vi "Gestion regulateurs EUROTHERM EPC3000.vi"() -> ()   [LabVIEW 2022 SP3]
uses:
  Enum/Enum r14.ctl
  Enum/Enum r7.ctl
  Variables globales/Variable glob generale.vi
  Variables globales/Variables glob EUROTHERM.vi
panel:
  in  "Onglets port COM":T1(tab)
  in  "1 COM reg":T2(array[cluster]) caption="COM1"
  in  "1 COM reg 2":T2(array[cluster])
  in  "1 COM reg 3":T2(array[cluster])
  in  "1 COM reg 4":T2(array[cluster])
  in  "1 COM reg 5":T2(array[cluster])
  out "Action":string="\nAction en cours\nVeuillez patienter"
  out "référence en sortie":refnum<vi>
  out "CUVE":string
  out "Fichier de rapport":path caption="Fichier rapport"
  out "Listing programmes":string
  out "Config + programmes":T3
  in  "Onglets actions":T4(tab)
  in  "Envoyer profil":bool
  in  "Onglet_Tinit":enum32{"Définir Tinit", "Acquérir Tinit"}(tab)
  in  "Val T ini":dbl=20.0 format="%#.1f"
  in  "Régulateur":u16(ring) items=["avant", "centre", "arrière"]
  in  "Début du profil":timestamp format="%<%H:%M:%S\n%A %d/%m/%y>T"
  in  "Charger profil":bool
  in  "Lire régulateur":bool
  in  "Sauvegarder profil":bool
  in  "Stop Régulation":bool
  in  "Start Régulation":bool
  in  "Test surveillance reg":bool caption="Accès par mot de passe"
  in  "Lire les alarmes":bool
  in  "Modifier les alarmes":bool
  in  "Alarme haute":dbl caption="Alarme haute (°C)" format="%#.1f"
  in  "Alarme basse":dbl caption="Alarme basse (°C)" format="%#.1f"
  in  "stop":bool
  out "Profil":cluster{"Y":dbl[], "Y":dbl[]}[](graph)
  out "Type de fin":string
  # "gestion des régulateurs EPC3000\n(PROTOCOLE MODBUS)"
  # "Ce logiciel et les informations qu'il contient, sont la propriété de l’IAS et ne peuvent être diffusés sans l’autorisation de la Station d’étalonnage"
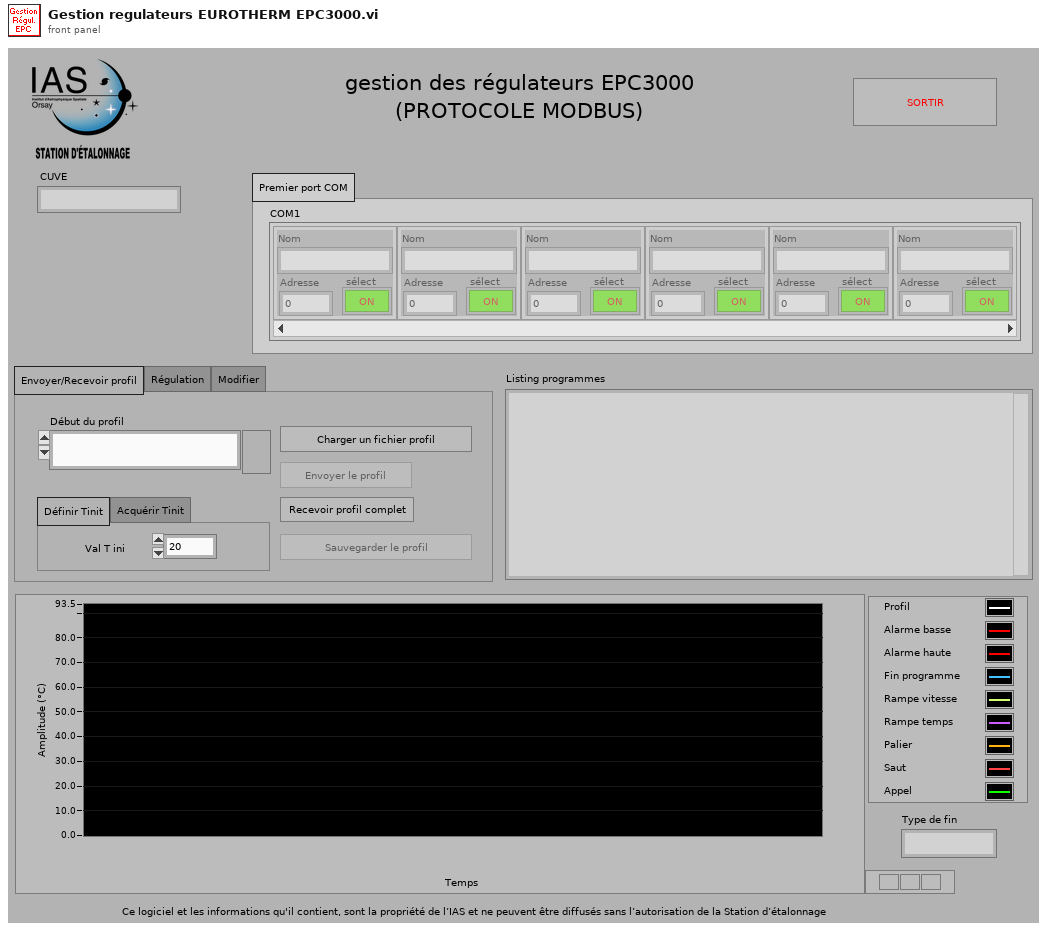
[diagram p1: front panel]
types:
  T1 = enum32{"Premier port COM", "Deuxième port COM", "Troisième port COM", "Quatrième port COM", "Cinquième port COM"}
  T2 = cluster{"Nom":string, "Adresse":u8, "sélect":bool}[]
  T3 = cluster{"config":cluster{"key":string, "value":dbl}[], "Prog 1 en sortie":cluster{string, dbl}[][], "Prog 2 en sortie":cluster{string, dbl}[][], "Prog 3 en sortie":cluster{string, dbl}[][], "Prog 4 en sortie":cluster{string, dbl}[][], "Prog 5 en sortie":cluster{string, dbl}[][], "Prog 6 en sortie":cluster{string, dbl}[][], "Prog 7 en sortie":cluster{string, dbl}[][], "Prog 8 en sortie":cluster{string, dbl}[][], "Prog 9 en sortie":cluster{string, dbl}[][], "Prog 10 en sortie":cluster{string, dbl}[][]}
  T4 = enum32{"Envoyer/Recevoir profil", "Régulation", "Modifier"}
  T5 = enum32{"Invalid", "Standard", "Closed", "Hidden", "Minimized", "Maximized"}
  T6 = cluster{cluster{"key":string, "value":i32}[], "Programme en sortie":cluster{string, dbl}[][], "Programme en sortie":cluster{string, dbl}[][], "Programme en sortie":cluster{string, dbl}[][], "Programme en sortie":cluster{string, dbl}[][], "Programme en sortie 2":cluster{string, dbl}[][], "Programme en sortie 3":cluster{string, dbl}[][], "Programme en sortie 4":cluster{string, dbl}[][], "Programme en sortie 5":cluster{string, dbl}[][], "Programme en sortie 6":cluster{string, dbl}[][], "Programme en sortie 7":cluster{string, dbl}[][]}
  T7 = enum8{"Enabled", "Disabled", "Disabled and Grayed Out"}
  T8 = typedef "Enum r14.ctl" = enum16{"RUN ?", "Arrêter ?", "Arrêt", "envoi profil", "fin"}
  T9 = typedef "Enum r7.ctl" = enum16{"validation liste", "réception profils", "validation RUN", "fin"}
  T10 = cluster{"1 COM reg":cluster{"Nom":string, "Adresse":u8, "sélect":bool}[]}[]
  T11 = cluster{"1 COM reg":cluster{"Nom":string, "Adresse":u8, "sélect":bool}[]}
  T12 = cluster{"config":cluster{"key":string, "value":dbl}[], "Prog 1":cluster{string, dbl}[][], "Prog 2":cluster{string, dbl}[][], "Prog 3":cluster{string, dbl}[][], "Prog 4":cluster{string, dbl}[][], "Prog 5":cluster{string, dbl}[][], "Prog 6":cluster{string, dbl}[][], "Prog 7":cluster{string, dbl}[][], "Prog 8":cluster{string, dbl}[][], "Prog 9":cluster{string, dbl}[][], "Prog 10":cluster{string, dbl}[][]}
  T13 = cluster{"Tempé. max":dbl, "Tempé. min":dbl, "Temps max":dbl, "Temps min":dbl}
  T14 = cluster{"Noms voies select acqui 1COM":string[]}[]
  T15 = cluster{"Ev_Saut":dbl[], "Ev_Palier":dbl[], "Ev_Rampe_vitesse":dbl[], "Ev_Rampe_temps":dbl[], "Ev_Appel":dbl[], "Ev_Fin":dbl[], "T_Fin":dbl[], "T_Appel":dbl[], "T_Rampe_temps":dbl[], "T_Rampe_vitesse":dbl[], "T_Palier":dbl[], "T_Saut":dbl[], "Type de fin":string}
  T16 = typedef "Commande Choix arret reg.ctl" = u16
  T17 = cluster{"Programmation configuration":cluster{"Command (PV)":string, dbl}[], "Programme 1":cluster{"chaîne o":string, "Received Value":dbl}[][], "Programme 2":cluster{"chaîne o":string, "Received Value":dbl}[][], "Programme 3":cluster{"chaîne o":string, "Received Value":dbl}[][], "Programme 4":cluster{"chaîne o":string, "Received Value":dbl}[][], "Programme 5":cluster{"chaîne o":string, "Received Value":dbl}[][], "Programme 6":cluster{"chaîne o":string, "Received Value":dbl}[][], "Programme 7":cluster{"chaîne o":string, "Received Value":dbl}[][], "Programme 8":cluster{"chaîne o":string, "Received Value":dbl}[][], "Programme 9":cluster{"chaîne o":string, "Received Value":dbl}[][], "Programme 10":cluster{"chaîne o":string, "Received Value":dbl}[][]}
  T18 = cluster{"config":cluster{"key":string, "value":dbl}[], "Programme_sortie":cluster{"chaîne":string, "Valeur":dbl}[][], "Programme_sortie":cluster{"chaîne":string, "Valeur":dbl}[][], "Programme_sortie":cluster{"chaîne":string, "Valeur":dbl}[][], "Programme_sortie":cluster{"chaîne":string, "Valeur":dbl}[][], "Programme_sortie":cluster{"chaîne":string, "Valeur":dbl}[][], "Programme_sortie":cluster{"chaîne":string, "Valeur":dbl}[][], "Programme_sortie":cluster{"chaîne":string, "Valeur":dbl}[][], "Programme_sortie":cluster{"chaîne":string, "Valeur":dbl}[][], "Programme_sortie":cluster{"chaîne":string, "Valeur":dbl}[][], "Programme_sortie":cluster{"chaîne":string, "Valeur":dbl}[][]}
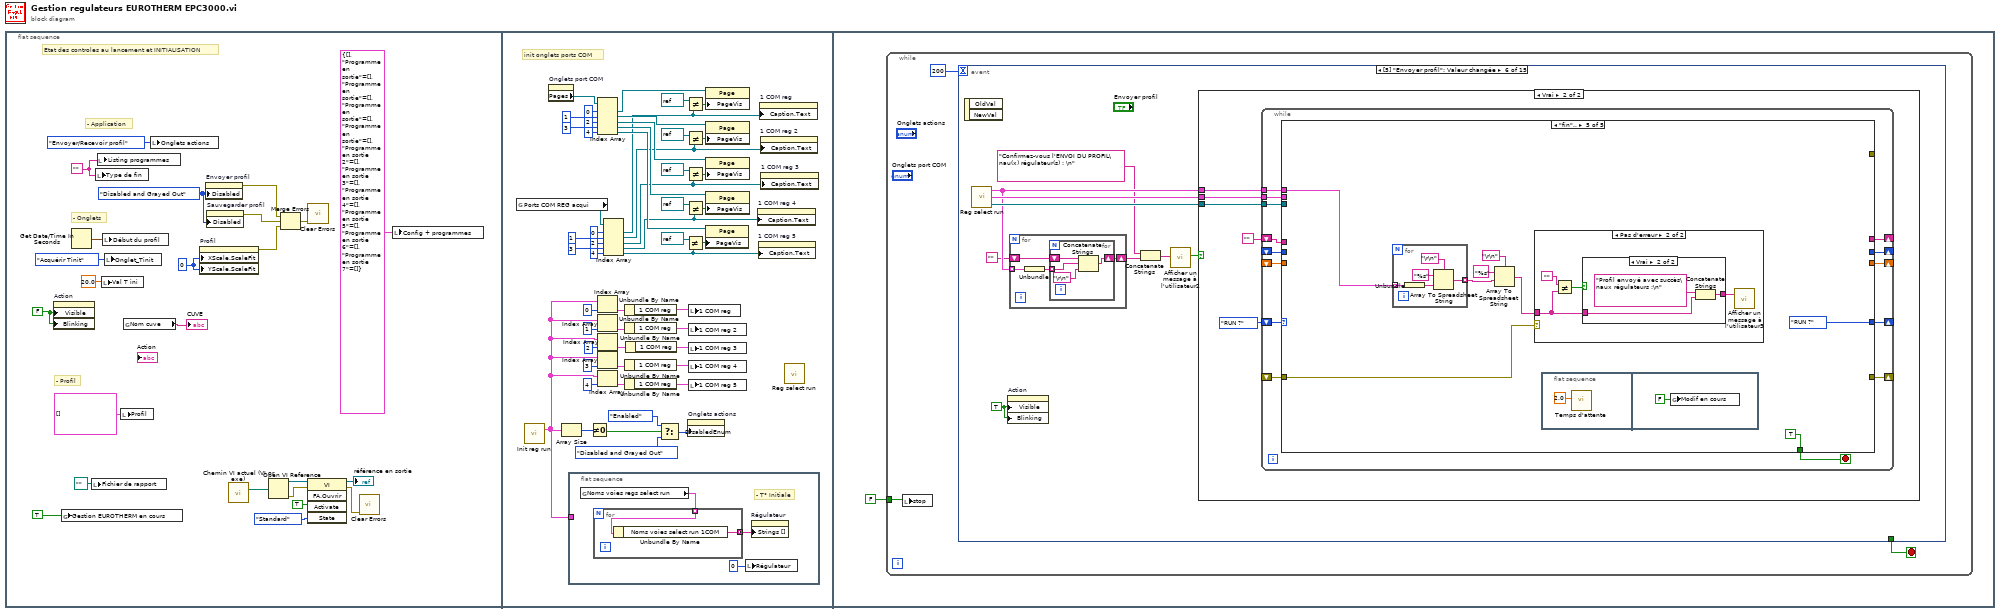
[diagram p0: block diagram]
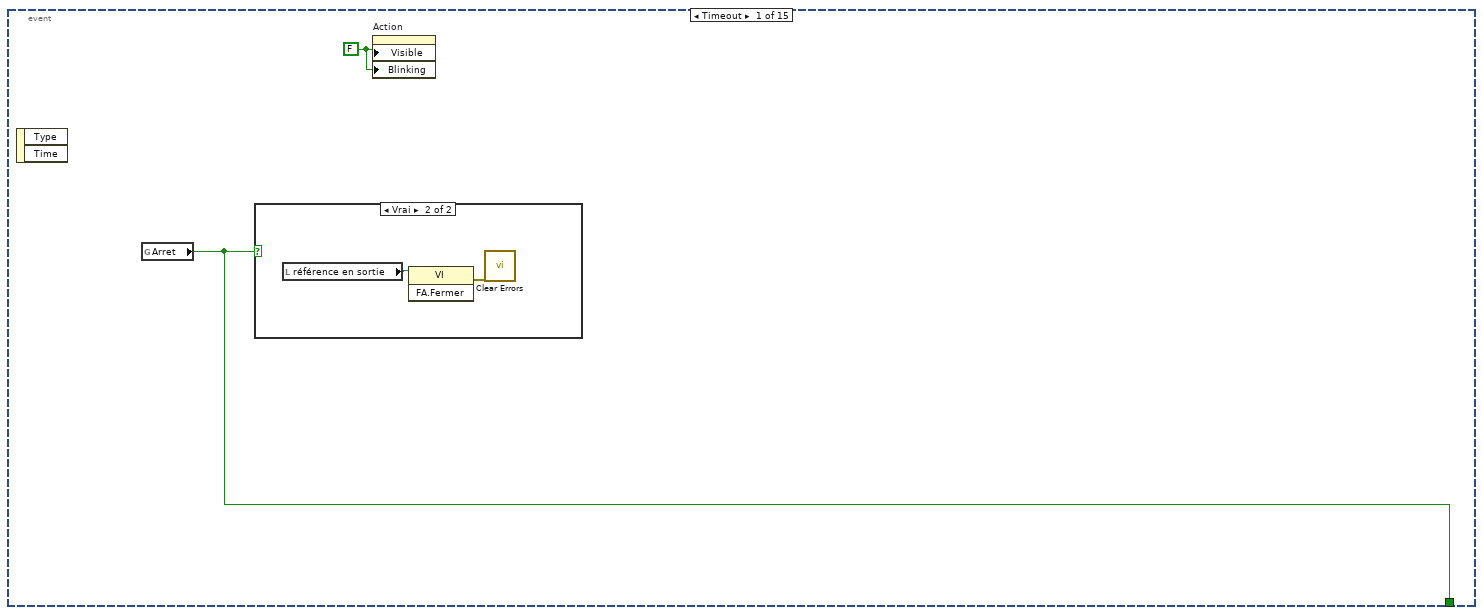
[diagram p2: hidden frame]
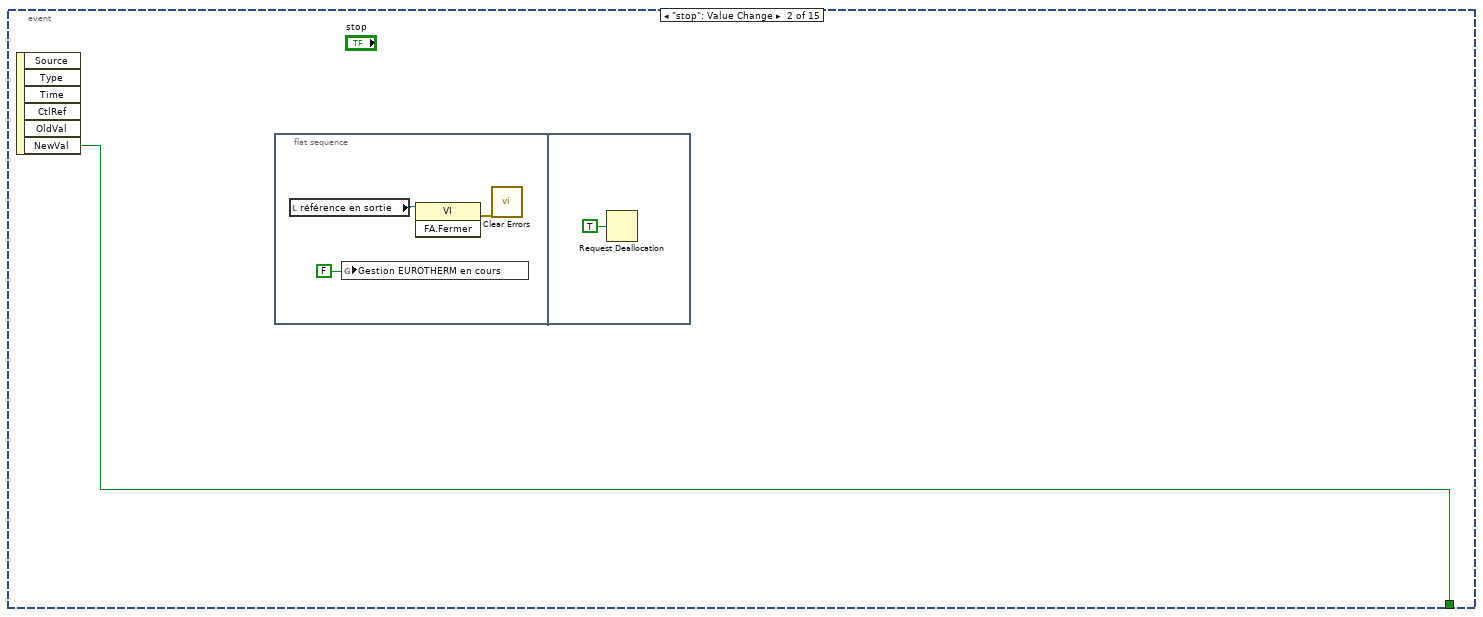
[diagram p4: hidden frame]
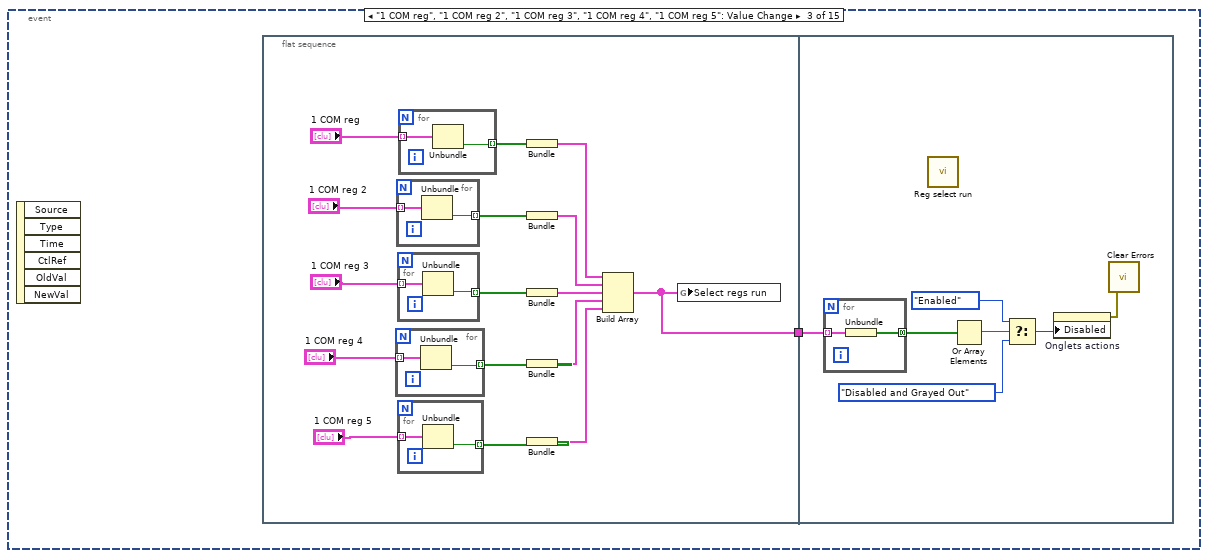
[diagram p5: hidden frame]
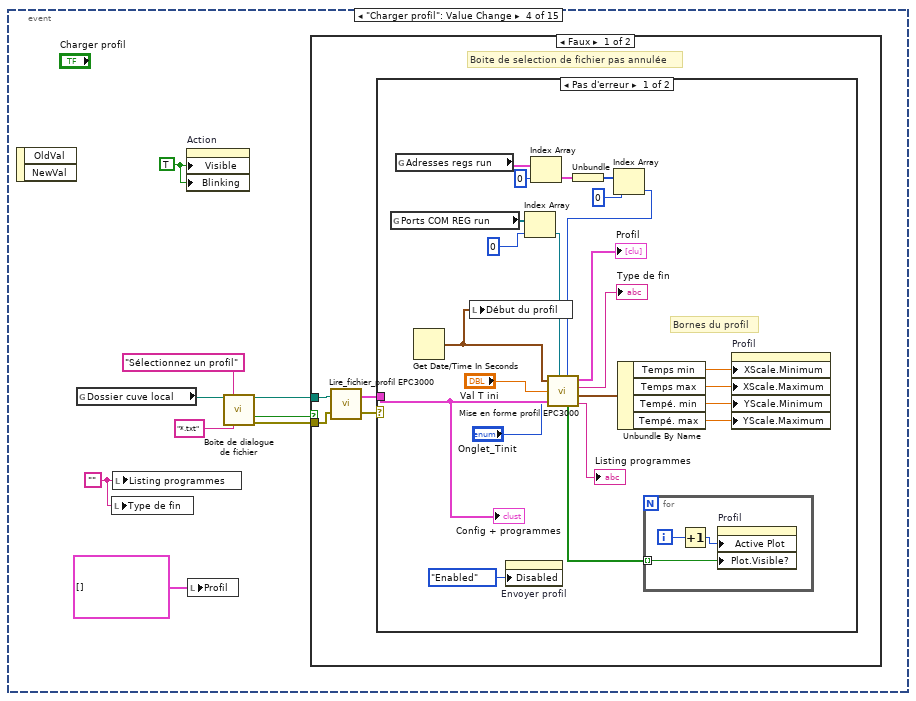
[diagram p6: hidden frame]
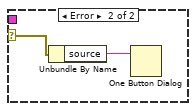
[diagram p7: hidden frame]
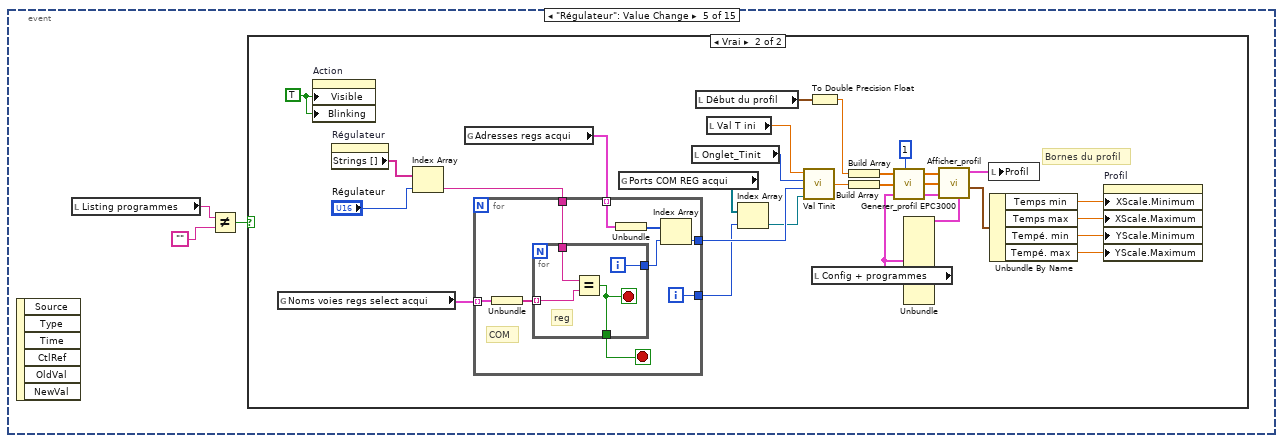
[diagram p9: hidden frame]
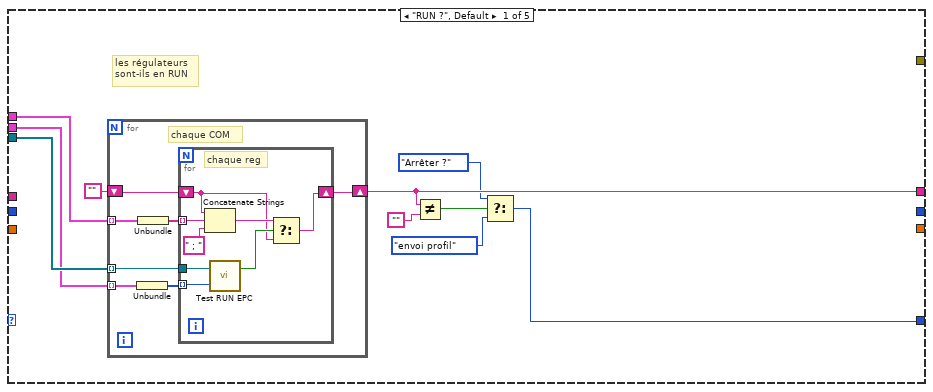
[diagram p12: hidden frame]
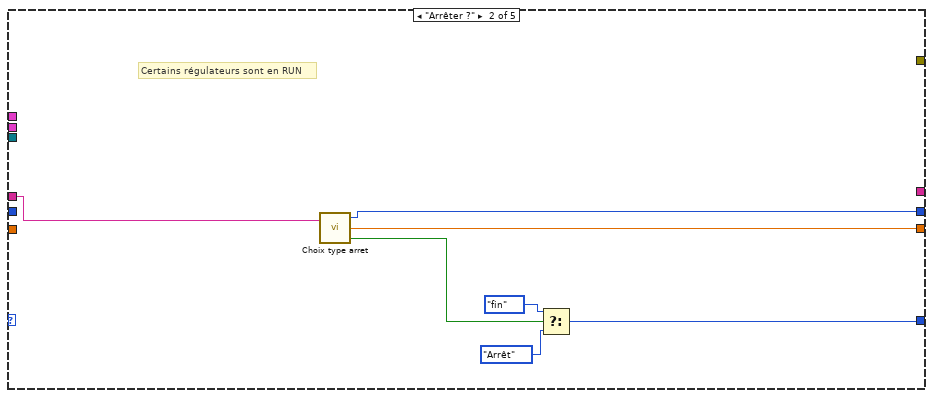
[diagram p13: hidden frame]
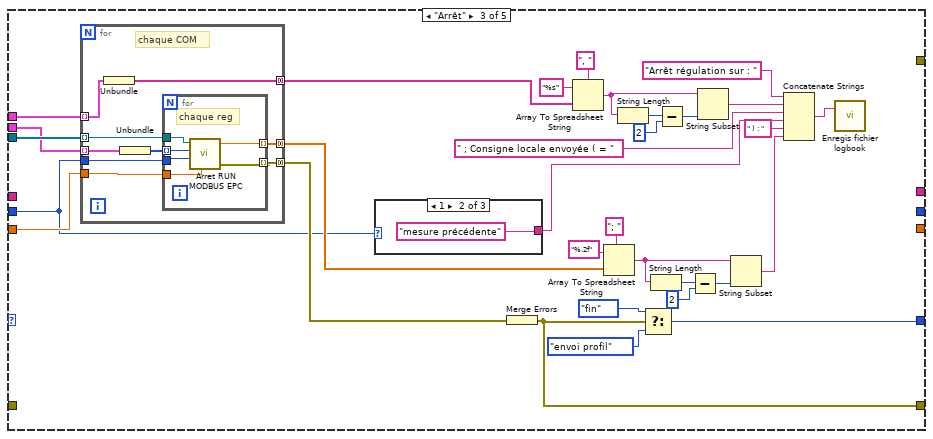
[diagram p14: hidden frame]
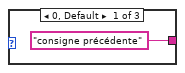
[diagram p15: hidden frame]
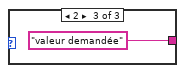
[diagram p16: hidden frame]
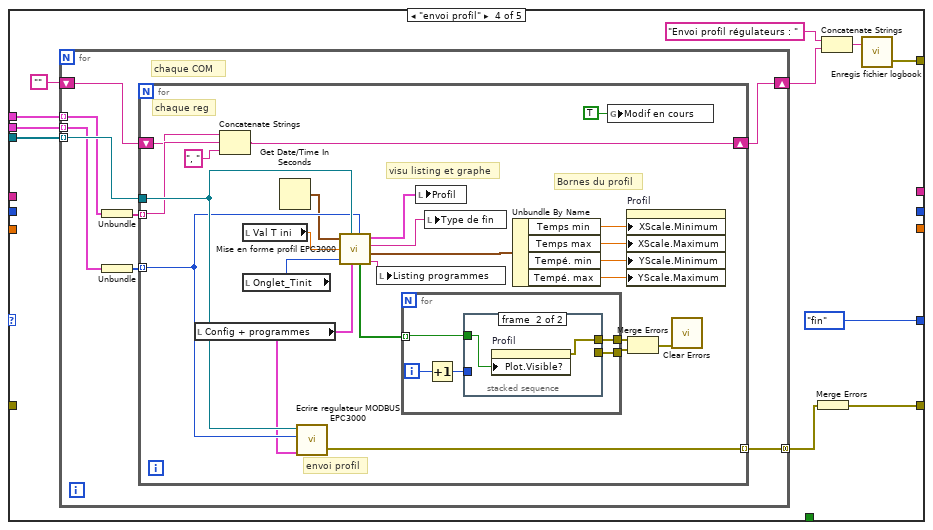
[diagram p17: hidden frame]
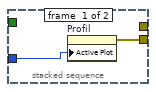
[diagram p18: hidden frame]
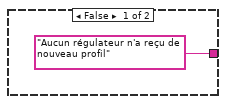
[diagram p20: hidden frame]
diagram:
  n1 = flat-sequence {
    frame #0 {
      w2 = T7."Disabled and Grayed Out" ("Désactivé")
      w3 = FALSE ("Visible")
      w22 = u8 0 ("Échelle des X.Ajuster l'échelle")
      w24 = ""
      # "- Onglets"
      # "- Profil"
      # "- Application"
      # "Etat des controles au lancement et INITIALISATION"
      n2 = property on="Action" class="Ch"("Visible"=w3, "Blinking"=w3) -> ()  [unwired: 2 in, 2 out]
      n3 = global write "Variable glob generale.vi" "Gestion EUROTHERM en cours"(TRUE ("Gestion reg en cours")) -> ()
      n4 = Get Date/Time In Seconds() -> (seconds since 1Jan1904=w21:timestamp)
      n5 = local write "Fichier de rapport"(path "" ("Fichier de rapport")) -> ()
      n6 = local write "Type de fin"(w24) -> ()
      n7 = local write "Listing programmes"(w24) -> ()
      n8 = local write "Val T ini"(20.0 ("Val_Tinit")) -> ()
      n9 = local write "Début du profil"(w21) -> ()
      n10 = local write "Onglet_Tinit"(enum32{"Définir Tinit", "Acquérir Tinit"}."Acquérir Tinit" ("Onglet_Tinit")) -> ()
      n11 = local write "Profil"(cluster{"Y":dbl[], "Y":dbl[]}[] [] ("Profil")) -> ()
      n12 = global read "Variable glob generale.vi" "Nom cuve"() -> (→"CUVE":string)
      n13 = local write "Onglets actions"(T4."Envoyer/Recevoir profil" ("Onglets actions")) -> ()
      n14 = property on="Profil" class="GraphXY (strict)"("XScale.ScaleFit"=w22, "YScale.ScaleFit"=w22) -> (error out=w15:errorcluster)  [unwired: 2 in, 1 out]
      n15 = property on="Envoyer profil" class="Bool"("Disabled"=w2) -> (error out=w16:errorcluster)  [unwired: 2 in, 1 out]
      n16 = property on="Sauvegarder profil" class="Bool"("Disabled"=w2) -> (error out=w14:errorcluster)  [unwired: 2 in, 1 out]
      n17 = call "Chemin VI actuel (VI or exe).vi"() -> ("Full Path to VI or executable"=w1:path)  [unwired: 14 in, 1 out]
      n18 = Open VI Reference(vi path=w1) -> (vi reference=w7:refnum<vi>, error out=w9:errorcluster)  [unwired: 5 in]
      n19 = Merge Errors(w16, w14, w15) -> (w13:errorcluster)
      n20 = invoke class="VI" method="FA.Ouvrir"(reference=w7, error in=w9, "Activate"=TRUE ("Activer ?"), "State"=T5."Standard" ("État")) -> (reference out=→"référence en sortie":refnum<vi>, error out=w10:errorcluster)  [unwired: 1 in, 3 out]
      n21 = call <vilib>:"Clear Errors.vi"("error in (no error)"=w13) -> ()  [unwired: 5 in, 2 out]
      n22 = call <vilib>:"Clear Errors.vi"("error in (no error)"=w10) -> ()  [unwired: 5 in, 2 out]
      n23 = local write "Config + programmes"(T6 {[], "Programme en sortie"=[], "Programme en sortie"=[], "Programme en sortie"=[], "Programme en sortie"=[], "Programme en sortie 2"=[], "Programme en sortie 3"=[], "Programme en sortie 4"=[], "Programme en sortie 5"=[], "Programme en sortie 6"=[], "Programme en sortie 7"=[]} ("Config + programmes")) -> ()
    }
    frame #1 {
      # "init onglets ports COM"
      n24 = global read "Variables glob EUROTHERM.vi" "Ports COM REG acqui"() -> (w65:refnum<visa-resource-name>[])
      n25 = call "Init reg run.vi"() -> ("Rég acqui"=w30:T10)  [unwired: 3 in]
      n26 = property on="Onglets port COM" class="Onglet (strict)"() -> ("Pages"=w72:refnum<vi>[])  [unwired: 2 in, 2 out]
      n27 = Array Size(array=w30) -> (size(s)=w29:i32)
      n28 = flat-sequence {
        tunnel: w30 -> [_]
        frame #0 {
          # "- T° Initiale"
          n29 = global read "Variables glob EUROTHERM.vi" "Noms voies regs select run"() -> (w80:cluster{"Noms voies select run 1COM":string[]}[])
          n30 = for {
            tunnel: w80 -> [w82] mode=indexing
            tunnel: [w81] -> w79 mode=concatenating
            n31 = Unbundle By Name(w82) -> ("Noms voies select run 1COM"=w81:string[])
          }
          n32 = local write "Régulateur"(0) -> ()
          n33 = property on="Régulateur" class="MDér (strict)"("Strings []"=w79) -> ()  [unwired: 2 in, 2 out]
        }
      }
      n34 = Not Equal To 0?(x=w29) -> (x != 0?=w28:bool)
      n35 = Index Array(array=w30, index=0 ("indice")) -> (element=w49:T11)
      n36 = Index Array(array=w30, index=1 ("indice")) -> (element=w46:T11)
      n37 = Index Array(array=w30, index=3 ("indice")) -> (element=w40:T11)
      n38 = Index Array(array=w30, index=4 ("indice")) -> (element=w37:T11)
      n39 = Index Array(array=w72, index #1=0 ("indice"), index #2=1 ("indice"), index #3=2 ("indice"), index #4=3 ("indice"), index #5=4 ("indice")) -> (element #1=w71:refnum<vi>, element #2=w60:refnum<vi>, element #3=w53:refnum<vi>, element #4=w52:refnum<vi>, element #5=w51:refnum<vi>)
      n40 = Index Array(array=w30, index=2 ("indice")) -> (element=w43:T11)
      n41 = Index Array(array=w65, index #1=0 ("indice"), index #2=1 ("indice"), index #3=2 ("indice"), index #4=3 ("indice"), index #5=4 ("indice")) -> (element #1=w33:refnum<visa-resource-name>, element #2=w32:refnum<visa-resource-name>, element #3=w31:refnum<visa-resource-name>, element #4=w34:refnum<visa-resource-name>, element #5=w35:refnum<visa-resource-name>)
      n42 = Unbundle By Name(w49) -> ("1 COM reg"=w48:T2)
      n43 = Unbundle By Name(w46) -> ("1 COM reg"=w47:T2)
      n44 = Unbundle By Name(w40) -> ("1 COM reg"=w41:T2)
      n45 = Unbundle By Name(w37) -> ("1 COM reg"=w36:T2)
      n46 = Unbundle By Name(w43) -> ("1 COM reg"=w42:T2)
      n47 = Select(t=T7."Enabled" ("Désactivé"), s=w28, f=T7."Disabled and Grayed Out" ("Désactivé")) -> (s? t:f=w25:T7)
      n48 = Not Equal?(x=refnum<visa-resource-name> refnum, y=w35) -> (x != y?=w54:bool)
      n49 = Not Equal?(x=refnum<visa-resource-name> refnum, y=w33) -> (x != y?=w64:bool)
      n50 = Not Equal?(x=refnum<visa-resource-name> refnum, y=w32) -> (x != y?=w61:bool)
      n51 = Not Equal?(x=refnum<visa-resource-name> refnum, y=w31) -> (x != y?=w56:bool)
      n52 = Not Equal?(x=refnum<visa-resource-name> refnum, y=w34) -> (x != y?=w59:bool)
      n53 = property on="Onglets actions" class="Onglet (strict)"("DisabledEnum"=w25) -> ()  [unwired: 2 in, 2 out]
      n54 = local write "1 COM reg"(w48) -> ()
      n55 = local write "1 COM reg 2"(w47) -> ()
      n56 = local write "1 COM reg 3"(w42) -> ()
      n57 = local write "1 COM reg 4"(w41) -> ()
      n58 = local write "1 COM reg 5"(w36) -> ()
      n59 = property class="Page"(reference=w51, "PageVis"=w54) -> ()  [unwired: 1 in, 2 out]
      n60 = property class="Page"(reference=w71, "PageVis"=w64) -> ()  [unwired: 1 in, 2 out]
      n61 = property class="Page"(reference=w60, "PageVis"=w61) -> ()  [unwired: 1 in, 2 out]
      n62 = property class="Page"(reference=w53, "PageVis"=w56) -> ()  [unwired: 1 in, 2 out]
      n63 = property class="Page"(reference=w52, "PageVis"=w59) -> ()  [unwired: 1 in, 2 out]
      n64 = property on="1 COM reg 4" class="Tabl (strict)"("Caption.Text"=w34) -> ()  [unwired: 2 in, 2 out]
      n65 = property on="1 COM reg 5" class="Tabl (strict)"("Caption.Text"=w35) -> ()  [unwired: 2 in, 2 out]
      n66 = property on="1 COM reg" class="Tabl (strict)"("Caption.Text"=w33) -> ()  [unwired: 2 in, 2 out]
      n67 = property on="1 COM reg 2" class="Tabl (strict)"("Caption.Text"=w32) -> ()  [unwired: 2 in, 2 out]
      n68 = property on="1 COM reg 3" class="Tabl (strict)"("Caption.Text"=w31) -> ()  [unwired: 2 in, 2 out]
      n69 = call "Reg select run.vi"() -> ()  [unwired: 2 in, 3 out]
    }
    frame #2 {
      n70 = while {
        tunnel: FALSE ("stop") -> [w86]
        stop <- w84 stop-if-true
        n71 = local write "stop"(w86) -> ()
        n72 = event shown="[5] \"Envoyer profil\": Valeur changée" {
          selector: _ -> [_ _ _ _ _ _ _ _ _ _ _ _ _ _ _]
          dyn-events: _ -> [_ _ _ _ _ _ _ _ _ _ _ _ _ _ _]
          timeout: 200 -> [_ _ _ _ _ _ _ _ _ _ _ _ _ _ _]
          tunnel: [w88 w91 _ _ _ _ _ _ _ _ _ _ _ _ _] -> w84
          event Timeout {
            w87 = FALSE ("Visible")
            n73 = event-data() -> ()  [unwired: 1 in, 2 out]
            n74 = global read "Variable glob generale.vi" "Arret"() -> (w88:bool)
            n75 = case shown="Vrai" w88 {
              frame False {
              }
              frame True {
                n76 = local read "référence en sortie"() -> (w89:refnum<vi>)
                n77 = invoke class="VI" method="FA.Fermer"(reference=w89) -> (error out=w90:errorcluster)  [unwired: 2 in, 2 out]
                n78 = call <vilib>:"Clear Errors.vi"("error in (no error)"=w90) -> ()  [unwired: 5 in, 2 out]
              }
            }
            n79 = property on="Action" class="Ch"("Visible"=w87, "Blinking"=w87) -> ()  [unwired: 2 in, 2 out]
          }
          event "stop": Value Change {
            n80 = event-data() -> ("NewVal"=w91:bool)  [unwired: 1 in, 5 out]
            n81 = flat-sequence {
              frame #0 {
                n82 = local read "référence en sortie"() -> (w93:refnum<vi>)
                n83 = global write "Variable glob generale.vi" "Gestion EUROTHERM en cours"(FALSE ("Gestion reg en cours")) -> ()
                n84 = invoke class="VI" method="FA.Fermer"(reference=w93) -> (error out=w94:errorcluster)  [unwired: 2 in, 2 out]
                n85 = call <vilib>:"Clear Errors.vi"("error in (no error)"=w94) -> ()  [unwired: 5 in, 2 out]
              }
              frame #1 {
                n86 = Request Deallocation(TRUE ("flag")) -> ()
              }
            }
          }
          event "1 COM reg", "1 COM reg 2", "1 COM reg 3", "1 COM reg 4", "1 COM reg 5": Value Change {
            n87 = event-data() -> ()  [unwired: 1 in, 6 out]
            n88 = flat-sequence {
              tunnel: [w97] -> w96
              tunnel: w96 -> [w123]
              frame #0 {
                n89 = for {
                  tunnel: "1 COM reg 4" -> [w116] mode=indexing
                  tunnel: [w115] -> w101 mode=indexing
                  n90 = Unbundle(w116) -> ("sélect"=w115:bool)  [unwired: 2 out]
                }
                n91 = for {
                  tunnel: "1 COM reg 2" -> [w120] mode=indexing
                  tunnel: [w119] -> w105 mode=indexing
                  n92 = Unbundle(w120) -> ("sélect"=w119:bool)  [unwired: 2 out]
                }
                n93 = for {
                  tunnel: "1 COM reg 3" -> [w118] mode=indexing
                  tunnel: [w117] -> w103 mode=indexing
                  n94 = Unbundle(w118) -> ("sélect"=w117:bool)  [unwired: 2 out]
                }
                n95 = for {
                  tunnel: "1 COM reg 5" -> [w114] mode=indexing
                  tunnel: [w113] -> w99 mode=indexing
                  n96 = Unbundle(w114) -> ("sélect"=w113:bool)  [unwired: 2 out]
                }
                n97 = for {
                  tunnel: "1 COM reg" -> [w122] mode=indexing
                  tunnel: [w121] -> w107 mode=indexing
                  n98 = Unbundle(w122) -> ("sélect"=w121:bool)  [unwired: 2 out]
                }
                n99 = Bundle(w107) -> (w106:cluster{bool[]})  [unwired: 1 in]
                n100 = Bundle(w105) -> (w104:cluster{bool[]})  [unwired: 1 in]
                n101 = Bundle(w103) -> (w102:cluster{bool[]})  [unwired: 1 in]
                n102 = Bundle(w101) -> (w100:cluster{bool[]})  [unwired: 1 in]
                n103 = Bundle(w99) -> (w98:cluster{bool[]})  [unwired: 1 in]
                n104 = Build Array(w106, w104, w102, w100, w98) -> (w97:cluster{bool[]}[])
                n105 = global write "Variables glob EUROTHERM.vi" "Select regs run"(w97) -> ()
              }
              frame #1 {
                n106 = for {
                  tunnel: w123 -> [w131] mode=indexing
                  tunnel: [w130] -> w124 mode=concatenating
                  n107 = Unbundle(w131) -> (w130:bool[])
                }
                n108 = call "Reg select run.vi"() -> ()  [unwired: 2 in, 3 out]
                n109 = Or Array Elements(Boolean array=w124) -> (logical OR=w127:bool)
                n110 = Select(t=T7."Enabled" ("Désactivé"), s=w127, f=T7."Disabled and Grayed Out" ("Désactivé")) -> (s? t:f=w129:T7)
                n111 = property on="Onglets actions" class="Onglet (strict)"("Disabled"=w129) -> (error out=w128:errorcluster)  [unwired: 2 in, 1 out]
                n112 = call <vilib>:"Clear Errors.vi"("error in (no error)"=w128) -> ()  [unwired: 5 in, 2 out]
              }
            }
          }
          event "Charger profil": Value Change {
            w133 = TRUE ("Visible")
            w134 = ""
            n113 = event-data() -> ()  [unwired: 1 in, 2 out]
            n114 = global read "Variable glob generale.vi" "Dossier cuve local"() -> (w136:path)
            n115 = local write "Type de fin"(w134) -> ()
            n116 = local write "Listing programmes"(w134) -> ()
            n117 = property on="Action" class="Ch"("Visible"=w133, "Blinking"=w133) -> ()  [unwired: 2 in, 2 out]
            n118 = local write "Profil"(cluster{"Y":dbl[], "Y":dbl[]}[] [] ("Profil")) -> ()
            n119 = call "Boîte de dialogue de fichier"("start path"=w136, "prompt"="Sélectionnez un profil", "pattern (all files)"="*.txt") -> ("selected path"=w137:path, "cancelled"=w138:bool, "error out"=w132:errorcluster)  [unwired: 9 in, 1 out]
            n120 = case shown="Faux" w138 {
              tunnel: w137 -> [w144 _]
              tunnel: w132 -> [w142 _]
              frame False {
                # "Boite de selection de fichier pas annulée"
                n121 = call "Lire_fichier_profil EPC3000.vi"("error in (no error)"=w142, "Chemin du fichier profil"=w144) -> ("error out"=w141:errorcluster, "Config + programmes"=w143:T12)
                n122 = case shown="Pas d'erreur" w141 {
                  selector: w141 -> [_ w172]
                  tunnel: w143 -> [w156 _]
                  frame No Error {
                    # "Bornes du profil"
                    n123 = global read "Variables glob EUROTHERM.vi" "Ports COM REG run"() -> (w153:refnum<visa-resource-name>[])
                    n124 = global read "Variables glob EUROTHERM.vi" "Adresses regs run"() -> (w150:cluster{"Adresses run 1COM reg":u16[]}[])
                    n125 = Get Date/Time In Seconds() -> (seconds since 1Jan1904=w154:timestamp)
                    n126 = local write "Début du profil"(w154) -> ()
                    n127 = property on="Envoyer profil" class="Bool"("Disabled"=T7."Enabled" ("Désactivé")) -> ()  [unwired: 2 in, 2 out]
                    n128 = Index Array(array=w153, index=0 ("indice")) -> (element=w151:refnum<visa-resource-name>)
                    n129 = Index Array(array=w150, index=0 ("indice")) -> (element=w148:cluster{"Adresses run 1COM reg":u16[]})
                    n130 = Unbundle(w148) -> ("Adresses run 1COM reg"=w147:u16[])
                    n131 = Index Array(array=w147, index=0 ("indice")) -> (element=w145:u16)
                    n132 = call "Mise en forme profil EPC3000.vi"("Début du profil"=w154, "Port COM run 1 REG"=w151, "Val T ini en entrée"="Val T ini", "Onglet_Tinit"="Onglet_Tinit", "Config + programmes"=w156, "adresse reg"=w145) -> ("Graphe XY"=→"Profil":cluster{"Y":dbl[], "Y":dbl[]}[], "Type de fin"=→"Type de fin":string, "Courbes à afficher"=w167:bool[], "Bornes profil"=w162:T13, "Listing_sortie"=→"Listing programmes":string)
                    n133 = Unbundle By Name(w162) -> ("Temps min"=w163:dbl, "Temps max"=w164:dbl, "Tempé. min"=w165:dbl, "Tempé. max"=w166:dbl)
                    n134 = for {
                      tunnel: w167 -> [w168] mode=indexing
                      i -> [w169]
                      n135 = Increment(x=w169) -> (x+1=w170:i32)
                      n136 = property on="Profil" class="GraphXY (strict)"("Active Plot"=w170, "Plot.Visible?"=w168) -> ()  [unwired: 2 in, 2 out]
                    }
                    n137 = property on="Profil" class="GraphXY (strict)"("XScale.Minimum"=w163, "XScale.Maximum"=w164, "YScale.Minimum"=w165, "YScale.Maximum"=w166) -> ()  [unwired: 2 in, 2 out]
                    "Config + programmes" <- w156
                  }
                  frame Error {
                    n138 = Unbundle By Name(w172) -> ("source"=w171:string)
                    n139 = One Button Dialog(message=w171) -> ()  [unwired: 1 in, 1 out]
                  }
                }
              }
              frame True {
                # "boite de dialogue fichier annulée"
              }
            }
          }
          event "Régulateur": Value Change {
            n140 = event-data() -> ()  [unwired: 1 in, 6 out]
            n141 = local read "Listing programmes"() -> (w175:string)
            n142 = Not Equal?(x=w175, y="") -> (x != y?=w173:bool)
            n143 = case shown="Vrai" w173 {
              frame False {
              }
              frame True {
                w179 = TRUE ("Visible")
                # "Bornes du profil"
                n144 = global read "Variables glob EUROTHERM.vi" "Noms voies regs select acqui"() -> (w183:T14)
                n145 = property on="Action" class="Ch"("Visible"=w179, "Blinking"=w179) -> ()  [unwired: 2 in, 2 out]
                n146 = property on="Régulateur" class="MDér (strict)"() -> ("Strings []"=w185:string[])  [unwired: 2 in, 2 out]
                n147 = Index Array(array=w185, index="Régulateur") -> (element=w182:string)
                n148 = global read "Variables glob EUROTHERM.vi" "Adresses regs acqui"() -> (w181:cluster{"Adresses acqui 1COM reg":u16[]}[])
                n149 = for {
                  tunnel: w183 -> [w213] mode=indexing
                  tunnel: w182 -> [w211]
                  tunnel: [w209] -> w177
                  tunnel: w181 -> [w208] mode=indexing
                  tunnel: [w205] -> w180
                  i -> [w209]
                  stop <- w210 stop-if-true
                  # "COM"
                  n150 = Unbundle(w213) -> ("Noms voies select acqui 1COM"=w212:string[])
                  n151 = for {
                    tunnel: w212 -> [w216] mode=indexing
                    tunnel: w211 -> [w217]
                    tunnel: [w215] -> w206
                    tunnel: [w214] -> w210
                    i -> [w215]
                    stop <- w214 stop-if-true
                    # "reg"
                    n152 = Equal?(x=w217, y=w216) -> (x = y?=w214:bool)
                  }
                  n153 = Unbundle(w208) -> ("Adresses acqui 1COM reg"=w207:u16[])
                  n154 = Index Array(array=w207, index=w206) -> (element=w205:u16)
                }
                n155 = global read "Variables glob EUROTHERM.vi" "Ports COM REG acqui"() -> (w178:refnum<visa-resource-name>[])
                n156 = local read "Onglet_Tinit"() -> (w196:enum32{"Définir Tinit", "Acquérir Tinit"})
                n157 = local read "Début du profil"() -> (w193:timestamp)
                n158 = local read "Val T ini"() -> (w195:dbl)
                n159 = Index Array(array=w178, index=w177) -> (element=w176:refnum<visa-resource-name>)
                n160 = call "Val Tinit.vi"("Port COM run 1 REG"=w176, "Adresse"=w180, "Onglet_Tinit"=w196, "Val T ini"=w195) -> ("Température"=w192:dbl)
                n161 = To Double Precision Float(number=w193) -> (double precision float=w194:dbl)
                n162 = local read "Config + programmes"() -> (w197:T3)
                n163 = Build Array(w194) -> (w188:dbl[])
                n164 = Build Array(w192) -> (w187:dbl[])
                n165 = call "Generer_profil EPC3000.vi"("Temps (s)"=w188, "Num_Prog"=u8 1, "Températures (°C)"=w187, "Programmes et config"=w197) -> ("Temps (s)"=w189:dbl[], "Températures (°C)"=w191:dbl[], "Evennements_sortie"=w190:T15)  [unwired: 1 in]
                n166 = Unbundle(w197) -> ("config"=w198:cluster{"key":string, "value":dbl}[])  [unwired: 10 out]
                n167 = call "Afficher_profil.vi"("Configuration"=w198, "Temps (s)"=w189, "Températures (°C)"=w191, "Evennements_entrée"=w190) -> ("Graphe XY"=w199:cluster{"Y":dbl[], "Y":dbl[]}[], "Bornes profil"=w204:T13)  [unwired: 2 out]
                n168 = local write "Profil"(w199) -> ()
                n169 = Unbundle By Name(w204) -> ("Temps min"=w203:dbl, "Temps max"=w202:dbl, "Tempé. min"=w201:dbl, "Tempé. max"=w200:dbl)
                n170 = property on="Profil" class="GraphXY (strict)"("XScale.Minimum"=w203, "XScale.Maximum"=w202, "YScale.Minimum"=w201, "YScale.Maximum"=w200) -> ()  [unwired: 2 in, 2 out]
              }
            }
          }
          event "Envoyer profil": Value Change {
            w226 = TRUE ("Visible")
            n171 = event-data() -> ()  [unwired: 1 in, 2 out]
            n172 = call "Reg select run.vi"() -> ("Noms sélect run"=w223:cluster{"Noms voies sélect run 1COM":string[]}[], "Adresses sélect run"=w224:cluster{"Adresses run 1COM reg":u8[]}[], "COM run"=w225:refnum<visa-resource-name>[])  [unwired: 2 in]
            n173 = property on="Action" class="Ch"("Visible"=w226, "Blinking"=w226) -> ()  [unwired: 2 in, 2 out]
            n174 = for {
              shift-right: [w230] -> w219
              shift-left: "" -> [w229]
              tunnel: w223 -> [w228] mode=indexing
              n175 = Unbundle(w228) -> ("Noms voies sélect run 1COM"=w227:string[])
              n176 = for {
                tunnel: w227 -> [w232] mode=indexing
                shift-right: [w234] -> w230
                shift-left: w229 -> [w233]
                n177 = Concatenate Strings(w233, w232, "\r\n") -> (w234:string)
              }
            }
            n178 = Concatenate Strings("Confirmez-vous l'ENVOI DU PROFIL\nau(x) régulateur(s) : \n", w219) -> (w218:string)
            n179 = call "Afficher un message à l'utilisateur2"("Message"=w218) -> ("OUI"=w221:bool)  [unwired: 9 in, 1 out]
            n180 = case shown="Vrai" w221 {
              tunnel: w225 -> [_ w239]
              tunnel: w224 -> [_ w238]
              tunnel: w223 -> [_ w237]
              frame False {
              }
              frame True {
                n181 = while {
                  tunnel: w239 -> [w253]
                  tunnel: w238 -> [w252]
                  tunnel: w237 -> [w251]
                  shift-right: [w247] -> _
                  shift-left: Enum_r14."RUN ?" ("Énum") -> [w250]
                  shift-right: [w249] -> _
                  shift-left: "" -> [w248]
                  shift-right: [w246] -> _
                  shift-left: _ -> [w245]
                  shift-right: [w243] -> _
                  shift-left: _ -> [w242]
                  shift-right: [w241] -> _
                  shift-left: _ -> [w240]
                  stop <- w244 stop-if-true
                  n182 = case shown="\"fin\".." w250 {
                    tunnel: w253 -> [w263 _ w316 w345 _]
                    tunnel: w252 -> [w262 _ w315 w344 _]
                    tunnel: w251 -> [w261 _ w308 w343 w392]
                    tunnel: [w259 _ _ _ _] -> w249
                    tunnel: w248 -> [_ w282 _ _ _]
                    tunnel: [w254 w283 w311 Enum_r14."fin" ("Énum") Enum_r14."RUN ?" ("Énum")] -> w247
                    tunnel: [_ w280 _ _ _] -> w246
                    tunnel: w245 -> [_ _ w289 _ _]
                    tunnel: [_ _ _ _ TRUE] -> w244
                    tunnel: [_ _ w310 w340 _] -> w243
                    tunnel: w242 -> [_ _ _ _ w387]
                    tunnel: [_ w279 _ _ _] -> w241
                    tunnel: w240 -> [_ _ w309 _ _]
                    tunnel: [_ _ _ w336 _] -> _
                    frame "RUN ?", Default {
                      # "les régulateurs\nsont-ils en RUN"
                      n183 = for {
                        tunnel: w263 -> [w270] mode=indexing
                        tunnel: w262 -> [w269] mode=indexing
                        tunnel: w261 -> [w267] mode=indexing
                        shift-right: [w264] -> w259
                        shift-left: "" -> [w265]
                        # "chaque COM"
                        n184 = Unbundle(w269) -> ("Adresses run 1COM reg"=w268:u8[])
                        n185 = Unbundle(w267) -> ("Noms voies sélect run 1COM"=w266:string[])
                        n186 = for {
                          tunnel: w268 -> [w277] mode=indexing
                          tunnel: w270 -> [w278]
                          tunnel: w266 -> [w272] mode=indexing
                          shift-right: [w274] -> w264
                          shift-left: w265 -> [w273]
                          # "chaque reg"
                          n187 = Concatenate Strings(w273, w272, " ; ") -> (w275:string)
                          n188 = call "Test RUN EPC.vi"("Adresse régulateur"=w277, "Port COM run 1 REG"=w278) -> ("En RUN"=w276:bool)  [unwired: 1 out]
                          n189 = Select(t=w275, s=w276, f=w273) -> (s? t:f=w274:string)
                        }
                      }
                      n190 = Not Equal?(x=w259, y="") -> (x != y?=w257:bool)
                      n191 = Select(t=Enum_r14."Arrêter ?" ("Énum"), s=w257, f=Enum_r14."envoi profil" ("Énum")) -> (s? t:f=w254:T8)
                    }
                    frame "Arrêter ?" {
                      # "Certains régulateurs sont en RUN"
                      n192 = call "Choix type arret.vi"("reg"=w282) -> ("Choix consigne locale : 2"=w280:T16, "Valeur"=w279:dbl, "annulé ?"=w281:bool)  [unwired: 1 in]
                      n193 = Select(t=Enum_r14."fin" ("Énum"), s=w281, f=Enum_r14."Arrêt" ("Énum")) -> (s? t:f=w283:T8)
                    }
                    frame "Arrêt" {
                      n194 = for {
                        tunnel: w316 -> [w328] mode=indexing
                        tunnel: w315 -> [w327] mode=indexing
                        tunnel: w289 -> [w325]
                        tunnel: [w324] -> w314 mode=concatenating
                        tunnel: w309 -> [w321]
                        tunnel: w308 -> [w323] mode=indexing
                        tunnel: [w322] -> w304 mode=concatenating
                        tunnel: [w320] -> w296 mode=concatenating
                        # "chaque COM"
                        n195 = Unbundle(w323) -> ("Noms voies sélect run 1COM"=w322:string[])
                        n196 = Unbundle(w327) -> ("Adresses run 1COM reg"=w326:u8[])
                        n197 = for {
                          tunnel: w328 -> [w334]
                          tunnel: w326 -> [w333] mode=indexing
                          tunnel: w325 -> [w331]
                          tunnel: [w332] -> w324 mode=indexing
                          tunnel: w321 -> [w330]
                          tunnel: [w329] -> w320 mode=indexing
                          # "chaque reg"
                          n198 = call "Arret RUN MODBUS EPC.vi"("Port COM run 1 REG"=w334, "Adresse"=w333, "Choix consigne locale :"=w331, "Valeur consigne"=w330) -> ("Consigne envoyée"=w329:dbl, "error out"=w332:errorcluster)  [unwired: 2 in]
                        }
                      }
                      n199 = case shown="1" w289 {
                        tunnel: ["consigne précédente" "mesure précédente" "valeur demandée"] -> w287
                        frame 0, Default {
                        }
                        frame 1 {
                        }
                        frame 2 {
                        }
                      }
                      n200 = Merge Errors(w314) -> (w310:errorcluster)
                      n201 = Array To Spreadsheet String(delimiter (Tab)=", " ("séparateur (Tabulation)"), array=w304, 3:"%s" ("chaîne de format")) -> (spreadsheet string=w291:string)
                      n202 = Array To Spreadsheet String(delimiter (Tab)="; " ("séparateur (Tabulation)"), array=w296, 3:"%.2f" ("chaîne de format")) -> (spreadsheet string=w301:string)
                      n203 = String Length(string=w291) -> (length=w292:i32)
                      n204 = Select(t=Enum_r14."fin" ("Énum"), s=w310, f=Enum_r14."envoi profil" ("Énum")) -> (s? t:f=w311:T8)
                      n205 = String Length(string=w301) -> (length=w300:i32)
                      n206 = Subtract(x=w292, y=2) -> (x-y=w293:i32)
                      n207 = Subtract(x=w300, y=2) -> (x-y=w299:i32)
                      n208 = String Subset(string=w291, length (rest)=w293) -> (substring=w290:string)  [unwired: 1 in]
                      n209 = String Subset(string=w301, length (rest)=w299) -> (substring=w288:string)  [unwired: 1 in]
                      n210 = Concatenate Strings("Arrêt régulation sur : ", w290, " ; Consigne locale envoyée ( = " ("chaîne"), w287, " ) : " ("chaîne"), w288) -> (w307:string)
                      n211 = call "Enregis fichier logbook.vi"("Chaîne"=w307) -> ()  [unwired: 2 in, 1 out]
                    }
                    frame "envoi profil" {
                      n212 = for {
                        tunnel: w345 -> [w353] mode=indexing
                        tunnel: w344 -> [w352] mode=indexing
                        tunnel: w343 -> [w350] mode=indexing
                        tunnel: [w349] -> w341 mode=concatenating
                        shift-right: [w346] -> w338
                        shift-left: "" -> [w347]
                        # "chaque COM"
                        n213 = Unbundle(w350) -> ("Noms voies sélect run 1COM"=w348:string[])
                        n214 = Unbundle(w352) -> ("Adresses run 1COM reg"=w351:u8[])
                        n215 = for {
                          tunnel: w348 -> [w375] mode=indexing
                          tunnel: w351 -> [w376] mode=indexing
                          tunnel: w353 -> [w377]
                          tunnel: [w374] -> w349 mode=indexing
                          shift-right: [w372] -> w346
                          shift-left: w347 -> [w373]
                          # "envoi profil"
                          # "Bornes du profil"
                          # "visu listing et graphe"
                          # "chaque reg"
                          n216 = local read "Config + programmes"() -> (w371:T3)
                          n217 = Concatenate Strings(w373, w375, ", ") -> (w372:string)
                          n218 = local read "Val T ini"() -> (w363:dbl)
                          n219 = local read "Onglet_Tinit"() -> (w369:enum32{"Définir Tinit", "Acquérir Tinit"})
                          n220 = Get Date/Time In Seconds() -> (seconds since 1Jan1904=w370:timestamp)
                          n221 = call "Ecrire regulateur MODBUS EPC3000.vi"("Config + programmes"=w371, "Adresse régulateur"=w376, "Port COM run 1 REG"=w377) -> ("error IO"=w374:errorcluster)  [unwired: 2 in]
                          n222 = call "Mise en forme profil EPC3000.vi"("Début du profil"=w370, "Port COM run 1 REG"=w377, "Val T ini en entrée"=w363, "Onglet_Tinit"=w369, "Config + programmes"=w371, "adresse reg"=w376) -> ("Graphe XY"=w365:cluster{"Y":dbl[], "Y":dbl[]}[], "Type de fin"=w366:string, "Courbes à afficher"=w364:bool[], "Bornes profil"=w367:T13, "Listing_sortie"=w368:string)
                          n223 = local write "Listing programmes"(w368) -> ()
                          n224 = for {
                            tunnel: w364 -> [w380] mode=indexing
                            tunnel: [w379] -> w360
                            tunnel: [w378] -> w361
                            i -> [w381]
                            n225 = Increment(x=w381) -> (x+1=w382:i32)
                            n226 = stacked-sequence {
                              tunnel: w380 -> [_ w386]
                              tunnel: w382 -> [w384 _]
                              tunnel: [w383 _] -> w378
                              tunnel: [_ w385] -> w379
                              frame #0 {
                                n227 = property on="Profil" class="GraphXY (strict)"("Active Plot"=w384) -> (error out=w383:errorcluster)  [unwired: 2 in, 1 out]
                              }
                              frame #1 {
                                n228 = property on="Profil" class="GraphXY (strict)"("Plot.Visible?"=w386) -> (error out=w385:errorcluster)  [unwired: 2 in, 1 out]
                              }
                            }
                          }
                          n229 = local write "Profil"(w365) -> ()
                          n230 = local write "Type de fin"(w366) -> ()
                          n231 = Unbundle By Name(w367) -> ("Temps min"=w356:dbl, "Temps max"=w357:dbl, "Tempé. min"=w358:dbl, "Tempé. max"=w359:dbl)
                          n232 = global write "Variables glob EUROTHERM.vi" "Modif en cours"(TRUE ("Modif en cours")) -> ()
                          n233 = property on="Profil" class="GraphXY (strict)"("XScale.Minimum"=w356, "XScale.Maximum"=w357, "YScale.Minimum"=w358, "YScale.Maximum"=w359) -> ()  [unwired: 2 in, 2 out]
                          n234 = Merge Errors(w360, w361) -> (w362:errorcluster)
                          n235 = call <vilib>:"Clear Errors.vi"("error in (no error)"=w362) -> ()  [unwired: 5 in, 2 out]
                        }
                      }
                      n236 = Merge Errors(w341) -> (w340:errorcluster)
                      n237 = Concatenate Strings("Envoi profil régulateurs : ", w338) -> (w337:string)
                      n238 = call "Enregis fichier logbook.vi"("Chaîne"=w337) -> ("sortie d'erreur"=w336:errorcluster)  [unwired: 2 in]
                    }
                    frame "fin".. {
                      n239 = for {
                        tunnel: w392 -> [w401] mode=indexing
                        tunnel: [w397] -> w389 mode=indexing
                        n240 = Unbundle(w401) -> ("Noms voies sélect run 1COM"=w400:string[])
                        n241 = Array To Spreadsheet String(delimiter (Tab)="\r\n", array=w400, 3:"%s" ("chaîne de format")) -> (spreadsheet string=w397:string)
                      }
                      n242 = Array To Spreadsheet String(delimiter (Tab)="\r\n", array=w389, 3:"%s" ("chaîne de format")) -> (spreadsheet string=w388:string)
                      n243 = case shown="Pas d'erreur" w387 {
                        tunnel: w388 -> [_ w404]
                        frame Error {
                        }
                        frame No Error {
                          n244 = Not Equal?(x="", y=w404) -> (x != y?=w403:bool)
                          n245 = case shown="Vrai" w403 {
                            tunnel: w404 -> [_ w407]
                            tunnel: ["Aucun régulateur n'a reçu de nouveau profil" w408] -> w402
                            frame False {
                            }
                            frame True {
                              n246 = Concatenate Strings("Profil envoyé avec succès\naux régulateurs :\n", w407) -> (w408:string)
                            }
                          }
                          n247 = call "Afficher un message à l'utilisateur3"("Message"=w402) -> ()  [unwired: 9 in, 2 out]
                        }
                      }
                      n248 = flat-sequence {
                        frame #0 {
                          n249 = call "Temps d'attente"("Delay Time (s)"=2.0) -> ()  [unwired: 10 in, 1 out]
                        }
                        frame #1 {
                          n250 = global write "Variables glob EUROTHERM.vi" "Modif en cours"(FALSE ("Modif en cours")) -> ()
                        }
                      }
                    }
                  }
                }
              }
            }
          }
          event "Lire régulateur": Value Change {
            w413 = ""
            w424 = TRUE ("Visible")
            n251 = event-data() -> ()  [unwired: 1 in, 6 out]
            n252 = call "Reg select run.vi"() -> ("Noms sélect run"=w411:cluster{"Noms voies sélect run 1COM":string[]}[], "Adresses sélect run"=w423:cluster{"Adresses run 1COM reg":u8[]}[], "COM run"=w415:refnum<visa-resource-name>[])  [unwired: 2 in]
            n253 = property on="Action" class="Ch"("Visible"=w424, "Blinking"=w424) -> ()  [unwired: 2 in, 2 out]
            n254 = Index Array(array=w423, index=0 ("indice")) -> (element=w421:cluster{"Adresses run 1COM reg":u8[]})
            n255 = local write "Type de fin"(w413) -> ()
            n256 = local write "Listing programmes"(w413) -> ()
            n257 = Index Array(array=w411, index=0 ("indice")) -> (element=w418:cluster{"Noms voies sélect run 1COM":string[]})
            n258 = for {
              tunnel: w411 -> [w429] mode=indexing
              tunnel: [w428] -> w410 mode=concatenating
              n259 = Unbundle(w429) -> ("Noms voies sélect run 1COM"=w428:string[])
            }
            n260 = Unbundle By Name(w418) -> ("Noms voies sélect run 1COM"=w417:string[])
            n261 = Index Array(array=w415, index=0 ("indice")) -> (element=w414:refnum<visa-resource-name>)
            n262 = Unbundle By Name(w421) -> ("Adresses run 1COM reg"=w420:u8[])
            n263 = local write "Profil"(cluster{"Y":dbl[], "Y":dbl[]}[] [] ("Profil")) -> ()
            n264 = Array Size(array=w410) -> (size(s)=w427:i32)
            n265 = Equal?(x=1, y=w427) -> (x = y?=w425:bool)
            n266 = case shown="Vrai" w425 {
              tunnel: w417 -> [_ w443]
              tunnel: w420 -> [_ w442]
              tunnel: w414 -> [_ w440]
              frame False {
                w430 = T7."Disabled and Grayed Out" ("Désactivé")
                n267 = property on="Sauvegarder profil" class="Bool"("Disabled"=w430) -> (error out=w433:errorcluster)  [unwired: 2 in, 1 out]
                n268 = property on="Envoyer profil" class="Bool"("Disabled"=w430) -> (error out=w432:errorcluster)  [unwired: 2 in, 1 out]
                n269 = Merge Errors(w433, w432) -> (w431:errorcluster)
                n270 = call <vilib>:"Clear Errors.vi"("error in (no error)"=w431) -> ()  [unwired: 5 in, 2 out]
                n271 = One Button Dialog(message="Vous ne pouvez lire qu'un régulateur à la fois") -> ()  [unwired: 1 in, 1 out]
              }
              frame True {
                # "Ok : un seul reg sélectionné"
                n272 = property on="Régulateur" class="MDér (strict)"() -> ("Strings []"=w438:string[])  [unwired: 2 in, 2 out]
                n273 = Index Array(array=w443) -> (element=w437:string)  [unwired: 1 in]
                n274 = Index Array(array=w442, index=0 ("indice")) -> (element=w439:u8)
                n275 = Search 1D Array(1D array=w438, element=w437, start index (0)=0 ("indice de départ (0)")) -> (index of element=w435:i32)
                n276 = local write "Régulateur"(w435) -> ()
                n277 = call "Lire regulateur MODBUS EPC3000.vi"("Adresse régulateur"=w439, "Port COM run 1 REG"=w440) -> ("error out"=w444:errorcluster, "Config + Programmes"=w445:T17)  [unwired: 2 in]
                n278 = case shown="Pas d'erreur" w444 {
                  selector: w444 -> [w447 _]
                  tunnel: w445 -> [_ w448]
                  tunnel: w439 -> [_ w449]
                  tunnel: w437 -> [_ w464]
                  tunnel: w440 -> [_ w450]
                  frame Error {
                    n279 = Unbundle By Name(w447) -> ("source"=w446:string)
                    n280 = One Button Dialog(message=w446) -> ()  [unwired: 1 in, 1 out]
                  }
                  frame No Error {
                    w460 = T7."Enabled" ("Désactivé")
                    # "Pas d'erreur de lecture du régulateur"
                    # "Affichage et activation des courbes"
                    n281 = call "Test RUN EPC.vi"("Adresse régulateur"=w449, "Port COM run 1 REG"=w450) -> ("En RUN"=w465:bool)  [unwired: 1 out]
                    n282 = local write "Config + programmes"(w448) -> ()
                    n283 = property on="Sauvegarder profil" class="Bool"("Disabled"=w460) -> (error out=w463:errorcluster)  [unwired: 2 in, 1 out]
                    n284 = property on="Envoyer profil" class="Bool"("Disabled"=w460) -> (error out=w462:errorcluster)  [unwired: 2 in, 1 out]
                    n285 = case shown="Vrai" w465 {
                      tunnel: [w471 w474] -> w451
                      tunnel: w464 -> [_ w473]
                      frame False {
                        # "Régulateur pas en RUN"
                        n286 = Get Date/Time In Seconds() -> (seconds since 1Jan1904=w471:timestamp)
                      }
                      frame True {
                        # "Régulateur en RUN"
                        n287 = local read "Fichier de rapport"() -> (w472:path)
                        n288 = call "lire fichier rapport.vi"("Nom du régulateur"=w473, "Fichier de rapport"=w472) -> ("début du profil"=w474:timestamp)
                      }
                    }
                    n289 = One Button Dialog(message="Lecture terminée avec succès") -> ()  [unwired: 1 in, 1 out]
                    n290 = Merge Errors(w463, w462) -> (w461:errorcluster)
                    n291 = call <vilib>:"Clear Errors.vi"("error in (no error)"=w461) -> ()  [unwired: 5 in, 2 out]
                    n292 = local read "Onglet_Tinit"() -> (w457:enum32{"Définir Tinit", "Acquérir Tinit"})
                    n293 = local read "Val T ini"() -> (w458:dbl)
                    n294 = local write "Début du profil"(w451) -> ()
                    n295 = call "Mise en forme profil EPC3000.vi"("Début du profil"=w451, "Port COM run 1 REG"=w450, "Val T ini en entrée"=w458, "Onglet_Tinit"=w457, "Config + programmes"=w448, "adresse reg"=w449) -> ("Graphe XY"=w455:cluster{"Y":dbl[], "Y":dbl[]}[], "Type de fin"=w454:string, "Courbes à afficher"=w456:bool[], "Bornes profil"=w453:T13, "Listing_sortie"=w452:string)
                    n296 = for {
                      tunnel: w456 -> [w476] mode=indexing
                      tunnel: [w475] -> w459
                      i -> [w477]
                      n297 = Increment(x=w477) -> (x+1=w478:i32)
                      n298 = property on="Profil" class="GraphXY (strict)"("Active Plot"=w478, "Plot.Visible?"=w476) -> (error out=w475:errorcluster)  [unwired: 2 in, 1 out]
                    }
                    n299 = local write "Listing programmes"(w452) -> ()
                    n300 = local write "Type de fin"(w454) -> ()
                    n301 = local write "Profil"(w455) -> ()
                    n302 = Unbundle By Name(w453) -> ("Temps min"=w469:dbl, "Temps max"=w468:dbl, "Tempé. min"=w467:dbl, "Tempé. max"=w466:dbl)
                    n303 = call <vilib>:"Clear Errors.vi"("error in (no error)"=w459) -> ()  [unwired: 5 in, 2 out]
                    n304 = property on="Profil" class="GraphXY (strict)"("XScale.Minimum"=w469, "XScale.Maximum"=w468, "YScale.Minimum"=w467, "YScale.Maximum"=w466) -> ()  [unwired: 2 in, 2 out]
                  }
                }
              }
            }
          }
          event "Sauvegarder profil": Value Change {
            n305 = event-data() -> ()  [unwired: 1 in, 6 out]
            n306 = global read "Variable glob generale.vi" "Dossier cuve local"() -> (w479:path)
            n307 = call "Boîte de dialogue de fichier2"("start path"=w479, "pattern (all files)"="*.txt") -> ("selected path"=w480:path, "cancelled"=w482:bool, "error out"=w484:errorcluster)  [unwired: 10 in, 1 out]
            n308 = Not(x=w482) -> (.not. x?=w483:bool)
            n309 = case shown="Vrai" w483 {
              tunnel: w480 -> [_ w505]
              tunnel: w484 -> [_ _]
              frame False {
              }
              frame True {
                # "Si pas annulé"
                # "On teste si les programmes sont vides. \nOn vérifie que les 4 programmes sont valides (Qu'ils contiennent au moins de segments, et que le dernier est une fin de programme).\nOn corrige si ce n'est pas le cas."
                n310 = local read "Config + programmes"() -> (w508:T3)
                n311 = Unbundle(w508) -> ("config"=w509:cluster{"key":string, "value":dbl}[], "Prog 1 en sortie"=w504:cluster{string, dbl}[][], "Prog 2 en sortie"=w503:cluster{string, dbl}[][], "Prog 3 en sortie"=w502:cluster{string, dbl}[][], "Prog 4 en sortie"=w501:cluster{string, dbl}[][], "Prog 5 en sortie"=w500:cluster{string, dbl}[][], "Prog 6 en sortie"=w499:cluster{string, dbl}[][], "Prog 7 en sortie"=w498:cluster{string, dbl}[][], "Prog 8 en sortie"=w497:cluster{string, dbl}[][], "Prog 9 en sortie"=w496:cluster{string, dbl}[][], "Prog 10 en sortie"=w495:cluster{string, dbl}[][])
                n312 = stacked-sequence {
                  tunnel: w504 -> [w511 _ _ _ _ _ _ _ _ _]
                  tunnel: w503 -> [_ w513 _ _ _ _ _ _ _ _]
                  tunnel: w502 -> [_ _ w515 _ _ _ _ _ _ _]
                  tunnel: w501 -> [_ _ _ w517 _ _ _ _ _ _]
                  tunnel: w500 -> [_ _ _ _ w519 _ _ _ _ _]
                  tunnel: w499 -> [_ _ _ _ _ w521 _ _ _ _]
                  tunnel: w498 -> [_ _ _ _ _ _ w523 _ _ _]
                  tunnel: w497 -> [_ _ _ _ _ _ _ w525 _ _]
                  tunnel: w496 -> [_ _ _ _ _ _ _ _ w527 _]
                  tunnel: w495 -> [_ _ _ _ _ _ _ _ _ w529]
                  tunnel: [w510 _ _ _ _ _ _ _ _ _] -> w494
                  tunnel: [_ w512 _ _ _ _ _ _ _ _] -> w493
                  tunnel: [_ _ w514 _ _ _ _ _ _ _] -> w492
                  tunnel: [_ _ _ w516 _ _ _ _ _ _] -> w491
                  tunnel: [_ _ _ _ w518 _ _ _ _ _] -> w490
                  tunnel: [_ _ _ _ _ w520 _ _ _ _] -> w489
                  tunnel: [_ _ _ _ _ _ w522 _ _ _] -> w488
                  tunnel: [_ _ _ _ _ _ _ w524 _ _] -> w487
                  tunnel: [_ _ _ _ _ _ _ _ w526 _] -> w486
                  tunnel: [_ _ _ _ _ _ _ _ _ w528] -> w485
                  frame #0 {
                    n313 = call "Verification_programme EPC3000.vi"("Programme_entrée"=w511) -> ("Programme_sortie"=w510:cluster{"chaîne":string, "Valeur":dbl}[][])
                  }
                  frame #1 {
                    n314 = call "Verification_programme EPC3000.vi"("Programme_entrée"=w513) -> ("Programme_sortie"=w512:cluster{"chaîne":string, "Valeur":dbl}[][])
                  }
                  frame #2 {
                    n315 = call "Verification_programme EPC3000.vi"("Programme_entrée"=w515) -> ("Programme_sortie"=w514:cluster{"chaîne":string, "Valeur":dbl}[][])
                  }
                  frame #3 {
                    n316 = call "Verification_programme EPC3000.vi"("Programme_entrée"=w517) -> ("Programme_sortie"=w516:cluster{"chaîne":string, "Valeur":dbl}[][])
                  }
                  frame #4 {
                    n317 = call "Verification_programme EPC3000.vi"("Programme_entrée"=w519) -> ("Programme_sortie"=w518:cluster{"chaîne":string, "Valeur":dbl}[][])
                  }
                  frame #5 {
                    n318 = call "Verification_programme EPC3000.vi"("Programme_entrée"=w521) -> ("Programme_sortie"=w520:cluster{"chaîne":string, "Valeur":dbl}[][])
                  }
                  frame #6 {
                    n319 = call "Verification_programme EPC3000.vi"("Programme_entrée"=w523) -> ("Programme_sortie"=w522:cluster{"chaîne":string, "Valeur":dbl}[][])
                  }
                  frame #7 {
                    n320 = call "Verification_programme EPC3000.vi"("Programme_entrée"=w525) -> ("Programme_sortie"=w524:cluster{"chaîne":string, "Valeur":dbl}[][])
                  }
                  frame #8 {
                    n321 = call "Verification_programme EPC3000.vi"("Programme_entrée"=w527) -> ("Programme_sortie"=w526:cluster{"chaîne":string, "Valeur":dbl}[][])
                  }
                  frame #9 {
                    n322 = call "Verification_programme EPC3000.vi"("Programme_entrée"=w529) -> ("Programme_sortie"=w528:cluster{"chaîne":string, "Valeur":dbl}[][])
                  }
                }
                n323 = Bundle("config"=w509, "Programme_sortie"=w494, "Programme_sortie"=w493, "Programme_sortie"=w492, "Programme_sortie"=w491, "Programme_sortie"=w490, "Programme_sortie"=w489, "Programme_sortie"=w488, "Programme_sortie"=w487, "Programme_sortie"=w486, "Programme_sortie"=w485) -> (w507:T18)  [unwired: 1 in]
                n324 = call "Enregistrer_fichier_profil EPC3000.vi"("Config + programmes"=w507, "Chemin du fichier profil"=w505) -> ("error out 2"=w506:errorcluster)  [unwired: 1 in, 1 out]
                n325 = case shown="Erreur" w506 {
                  selector: w506 -> [_ w531]
                  frame No Error {
                  }
                  frame Error {
                    n326 = Unbundle By Name(w531) -> ("source"=w530:string)
                    n327 = One Button Dialog(message=w530) -> ()  [unwired: 1 in, 1 out]
                  }
                }
              }
            }
          }
          event "Start Régulation": Value Change {
            n328 = event-data() -> ("NewVal"=w532:bool)  [unwired: 1 in, 5 out]
            n329 = case shown="Vrai" w532 {
              frame True {
                # "Régulation"
                n330 = call "Reg select run.vi"() -> ("Noms sélect run"=w536:cluster{"Noms voies sélect run 1COM":string[]}[])  [unwired: 2 in, 2 out]
                n331 = for {
                  shift-right: [w610] -> w533
                  shift-left: "" -> [w609]
                  tunnel: w536 -> [w608] mode=indexing
                  n332 = Unbundle(w608) -> ("Noms voies sélect run 1COM"=w607:string[])
                  n333 = for {
                    tunnel: w607 -> [w612] mode=indexing
                    shift-right: [w614] -> w610
                    shift-left: w609 -> [w613]
                    n334 = Concatenate Strings(w613, w612, "\r\n") -> (w614:string)
                  }
                }
                n335 = while {
                  shift-right: [w541] -> _
                  shift-left: Enum_r7."validation liste" ("Énum") -> [w542]
                  tunnel: w533 -> [w539]
                  shift-right: [w538] -> _
                  shift-left: _ -> [w537]
                  stop <- w540 stop-if-true
                  n336 = case shown="\"réception profils\"" w542 {
                    tunnel: [w544 w553 Enum_r7."fin" ("Énum") Enum_r7."validation liste" ("Énum")] -> w541
                    tunnel: [_ _ _ TRUE] -> w540
                    tunnel: w539 -> [w543 _ w584 _]
                    tunnel: [_ w551 _ _] -> w538
                    tunnel: w537 -> [_ _ w581 _]
                    frame "validation liste", Default {
                      n337 = Concatenate Strings("Demande de RUN sur les régulateurs suivants :\n", w543, "Les profils vont être affichés avant validation des RUN.") -> (w550:string)
                      n338 = call "Afficher un message à l'utilisateur"("Message"=w550) -> ("OUI"=w545:bool)  [unwired: 9 in, 1 out]
                      n339 = Select(t=Enum_r7."réception profils" ("Énum"), s=w545, f=Enum_r7."fin" ("Énum")) -> (s? t:f=w544:T9)
                    }
                    frame "réception profils" {
                      n340 = global read "Variable glob generale.vi" "Sous-dossier"() -> (w579:string)
                      n341 = global read "Variable glob generale.vi" "Dossier cuve local"() -> (w568:path)
                      n342 = global read "Variable glob generale.vi" "Nom manip"() -> (w573:string)
                      n343 = Get Date/Time In Seconds() -> (seconds since 1Jan1904=w567:timestamp)
                      n344 = String Length(string=w579) -> (length=w574:i32)
                      n345 = Get Date/Time String(seconds (now)=w567) -> (date string=w562:string)  [unwired: 2 in, 1 out]
                      n346 = Build Path(base path=w568, name or relative path=w573) -> (appended path=w578:path)
                      n347 = Greater?(x=w574, y=1) -> (0:w576:bool)
                      n348 = String Subset(string=w562, offset (0)=6, length (rest)=4 ("longueur (reste)")) -> (substring=w561:string)
                      n349 = Build Path(base path=w578, name or relative path=w579) -> (appended path=w580:path)
                      n350 = String Subset(string=w562, offset (0)=3, length (rest)=2 ("longueur (reste)")) -> (substring=w559:string)
                      n351 = Select(t=w580, s=w576, f=w578) -> (s? t:f=w577:path)
                      n352 = Concatenate Strings(w561, "\\" ("chaîne"), w559) -> (w558:string)
                      n353 = Build Path(base path=w577, name or relative path=w558) -> (appended path=w569:path)
                      n354 = global read "Variable glob generale.vi" "Commentaire"() -> (w570:string)
                      n355 = call "Creation_chemin.vi"("Répertoire de travail"=w569) -> ("Chemin du fichier"=w557:path)  [unwired: 1 in]
                      "Fichier de rapport" <- w557
                      n356 = call "RUN regulateur MODBUS EPC3000.vi"("Commentaires"=w570, "Fichier rapport"=w557) -> ("error out"=w572:errorcluster, "annulé"=w552:bool)
                      n357 = property on="Onglets actions" class="Onglet (strict)"("Disabled"=T7."Disabled and Grayed Out" ("Désactivé")) -> (error out=w556:errorcluster)  [unwired: 2 in, 1 out]
                      n358 = Unbundle By Name(w572) -> ("source"=w551:string)
                      n359 = call <vilib>:"Clear Errors.vi"("error in (no error)"=w556) -> ()  [unwired: 5 in, 2 out]
                      n360 = Select(t=Enum_r7."fin" ("Énum"), s=w552, f=Enum_r7."validation RUN" ("Énum")) -> (s? t:f=w553:T9)
                    }
                    frame "validation RUN" {
                      n361 = Equal?(x="", y=w581) -> (x = y?=w583:bool)
                      n362 = case shown="Vrai" w583 {
                        tunnel: [w587 w602] -> w586
                        tunnel: w584 -> [_ w588]
                        tunnel: w581 -> [w587 _]
                        frame False {
                        }
                        frame True {
                          n363 = Search and Replace String(replace all?=TRUE ("tout remplacer ? (F)"), input string=w588, search string="\r\n", replace string=", " ("chaîne de remplacement (\"\")")) -> (result string=w594:string)  [unwired: 4 in, 3 out]
                          n364 = global read "Variable glob generale.vi" "Nom cuve"() -> (w598:string)
                          n365 = Concatenate Strings("Profil démarré (RUN) sur les régulateurs :\n" ("chaîne"), w588) -> (w597:string)
                          n366 = Equal?(x=w598, y="SUN") -> (x = y?=w601:bool)
                          n367 = Concatenate Strings(w597, "\nPENSER Á  ACTIVER LA PUISSANCE\nET ALIMENTER LA BOUTEILLE LN2" ("chaîne")) -> (w595:string)
                          n368 = Concatenate Strings("Profil démarré (RUN) sur les régulateurs : " ("chaîne"), w594) -> (w593:string)
                          n369 = Select(t=w597, s=w601, f=w595) -> (s? t:f=w602:string)
                          n370 = call "Enregis fichier logbook.vi"("Chaîne"=w593) -> ()  [unwired: 2 in, 1 out]
                        }
                      }
                      n371 = call "Afficher un message à l'utilisateur4"("Message"=w586) -> ()  [unwired: 9 in, 2 out]
                    }
                    frame "fin" {
                      n372 = property on="Onglets actions" class="Onglet (strict)"("Disabled"=T7."Enabled" ("Désactivé")) -> (error out=w605:errorcluster)  [unwired: 2 in, 1 out]
                      n373 = call <vilib>:"Clear Errors.vi"("error in (no error)"=w605) -> ()  [unwired: 5 in, 2 out]
                    }
                  }
                }
              }
              frame False {
              }
            }
          }
          event "Stop Régulation": Value Change {
            n374 = event-data() -> ()  [unwired: 1 in, 6 out]
            n375 = global read "Variables glob EUROTHERM.vi" "Noms voies regs select run"() -> (w620:cluster{"Noms voies select run 1COM":string[]}[])
            n376 = for {
              shift-right: [w624] -> w615
              shift-left: "" -> [w623]
              tunnel: w620 -> [w622] mode=indexing
              n377 = Unbundle(w622) -> ("Noms voies select run 1COM"=w621:string[])
              n378 = for {
                tunnel: w621 -> [w626] mode=indexing
                shift-right: [w628] -> w624
                shift-left: w623 -> [w627]
                n379 = Concatenate Strings(w627, w626, "\r\n") -> (w628:string)
              }
            }
            n380 = call "Choix type arret.vi"("reg"=w615) -> ("Choix consigne locale : 2"=w616:T16, "Valeur"=w617:dbl, "annulé ?"=w618:bool)  [unwired: 1 in]
            n381 = case shown="Faux" w618 {
              tunnel: w617 -> [w648 _]
              tunnel: w616 -> [w633 _]
              tunnel: w615 -> [w647 _]
              frame False {
                n382 = global read "Variables glob EUROTHERM.vi" "Ports COM REG run"() -> (w650:refnum<visa-resource-name>[])
                n383 = global read "Variables glob EUROTHERM.vi" "Adresses regs run"() -> (w649:cluster{"Adresses run 1COM reg":u16[]}[])
                n384 = for {
                  tunnel: w650 -> [w659] mode=indexing
                  tunnel: w649 -> [w658] mode=indexing
                  tunnel: w633 -> [w656]
                  tunnel: w648 -> [w655]
                  tunnel: [w654] -> w641 mode=concatenating
                  # "Arrêt régulation"
                  n385 = Unbundle By Name(w658) -> ("Adresses run 1COM reg"=w657:u16[])
                  n386 = for {
                    tunnel: w659 -> [w663]
                    tunnel: w657 -> [w664] mode=indexing
                    tunnel: w656 -> [w662]
                    tunnel: w655 -> [w661]
                    tunnel: [w660] -> w654 mode=indexing
                    n387 = call "Arret RUN MODBUS EPC.vi"("Port COM run 1 REG"=w663, "Adresse"=w664, "Choix consigne locale :"=w662, "Valeur consigne"=w661) -> ("Consigne envoyée"=w660:dbl)  [unwired: 2 in, 1 out]
                  }
                }
                n388 = case shown="2" w633 {
                  tunnel: ["consigne précédente" "mesure précédente" "valeur demandée"] -> w631
                  frame 0, Default {
                  }
                  frame 1 {
                  }
                  frame 2 {
                  }
                }
                n389 = Array To Spreadsheet String(delimiter (Tab)="; " ("séparateur (Tabulation)"), array=w641, 3:"%.2f" ("chaîne de format")) -> (spreadsheet string=w638:string)
                n390 = Search and Replace String(replace all?=TRUE ("tout remplacer ? (F)"), input string=w647, search string="\r\n", replace string=", ") -> (result string=w642:string)  [unwired: 4 in, 3 out]
                n391 = String Length(string=w638) -> (length=w636:i32)
                n392 = Subtract(x=w636, y=2) -> (x-y=w634:i32)
                n393 = String Subset(string=w638, length (rest)=w634) -> (substring=w637:string)  [unwired: 1 in]
                n394 = Concatenate Strings("Arrêt régulation sur : ", w642, " ; Consigne locale envoyée ( = " ("chaîne"), w631, " ) : " ("chaîne"), w637) -> (w629:string)
                n395 = call "Enregis fichier logbook.vi"("Chaîne"=w629) -> ()  [unwired: 2 in, 1 out]
              }
              frame True {
                # "demande annulée"
              }
            }
          }
          event "Lire les alarmes": Value Change {
            w673 = TRUE ("Visible")
            n396 = event-data() -> ()  [unwired: 1 in, 6 out]
            n397 = call "Reg select run.vi"() -> ("Adresses sélect run"=w666:cluster{"Adresses run 1COM reg":u8[]}[], "COM run"=w668:refnum<visa-resource-name>[])  [unwired: 2 in, 1 out]
            n398 = for {
              tunnel: w666 -> [w678] mode=indexing
              tunnel: [w677] -> w665 mode=concatenating
              n399 = Unbundle(w678) -> ("Adresses run 1COM reg"=w677:u8[])
            }
            n400 = Index Array(array=w666, index=0 ("indice")) -> (element=w671:cluster{"Adresses run 1COM reg":u8[]})
            n401 = Array Size(array=w665) -> (size(s)=w676:i32)
            n402 = Unbundle By Name(w671) -> ("Adresses run 1COM reg"=w670:u8[])
            n403 = property on="Action" class="Ch"("Visible"=w673, "Blinking"=w673) -> ()  [unwired: 2 in, 2 out]
            n404 = Equal?(x=1, y=w676) -> (x = y?=w674:bool)
            n405 = Index Array(array=w668, index=0 ("indice")) -> (element=w667:refnum<visa-resource-name>)
            n406 = case shown="Vrai" w674 {
              tunnel: w670 -> [_ w681]
              tunnel: w667 -> [_ w680]
              frame False {
                n407 = One Button Dialog(message="Vous ne pouvez lire qu'un régulateur à la fois") -> ()  [unwired: 1 in, 1 out]
              }
              frame True {
                # "Un seul régulateur sélectionné"
                n408 = Index Array(array=w681) -> (element=w685:u8)  [unwired: 1 in]
                n409 = call "Lire_la_configuration.vi"("Port COM run 1 REG"=w680, "Adresse rég"=w685) -> ("AL haute sécu"=w684:dbl, "AL basse sécu"=w683:dbl, "error out"=w682:errorcluster)  [unwired: 1 in, 1 out]
                n410 = case shown="Pas d'erreur" w682 {
                  selector: w682 -> [_ w689]
                  tunnel: w684 -> [w686 _]
                  tunnel: w683 -> [w687 _]
                  frame No Error {
                    n411 = local write "Alarme basse"(w687) -> ()
                    n412 = local write "Alarme haute"(w686) -> ()
                  }
                  frame Error {
                    n413 = Unbundle By Name(w689) -> ("source"=w688:string)
                    n414 = One Button Dialog(message=w688) -> ()  [unwired: 1 in, 1 out]
                  }
                }
              }
            }
          }
          event "Modifier les alarmes": Value Change {
            w696 = TRUE ("Visible")
            n415 = event-data() -> ()  [unwired: 1 in, 6 out]
            n416 = property on="Action" class="Ch"("Visible"=w696, "Blinking"=w696) -> ()  [unwired: 2 in, 2 out]
            n417 = call "Reg select run.vi"() -> ("Noms sélect run"=w695:cluster{"Noms voies sélect run 1COM":string[]}[])  [unwired: 2 in, 2 out]
            n418 = for {
              shift-right: [w716] -> w690
              shift-left: "" -> [w715]
              tunnel: w695 -> [w714] mode=indexing
              n419 = Unbundle(w714) -> ("Noms voies sélect run 1COM"=w713:string[])
              n420 = for {
                tunnel: w713 -> [w717] mode=indexing
                shift-right: [w720] -> w716
                shift-left: w715 -> [w719]
                n421 = Concatenate Strings(w719, w717, "\r\n") -> (w720:string)
              }
            }
            n422 = Concatenate Strings("Êtes-vous sur de vouloir modifier les ALARMES\ndes régulateurs :\n" ("message"), w690) -> (w692:string)
            n423 = call "Afficher un message à l'utilisateur6"("Message"=w692) -> ("OUI"=w691:bool)  [unwired: 9 in, 1 out]
            n424 = case shown="Vrai" w691 {
              tunnel: w690 -> [_ w711]
              frame False {
              }
              frame True {
                n425 = Search and Replace String(replace all?=TRUE ("tout remplacer ? (F)"), input string=w711, search string="\r\n", replace string=", ") -> (result string=w706:string)  [unwired: 4 in, 3 out]
                n426 = local read "Fichier de rapport"() -> (w712:path)
                n427 = Number To Fractional String(number="Alarme basse", precision (6)=i16 2 ("précision (6)")) -> (F-format string=w700:string)  [unwired: 2 in]
                n428 = Number To Fractional String(number="Alarme haute", precision (6)=i16 2 ("précision (6)")) -> (F-format string=w697:string)  [unwired: 2 in]
                n429 = Concatenate Strings("Alarmes modifiées sur régulateurs : ", w706, ". Nouvelles alarmes envoyées : haute = ", w697, ", basse = ", w700) -> (w703:string)
                n430 = call "Envoi alarmes MODBUS EPC.vi"("Alarme haute"="Alarme haute", "Alarme basse"="Alarme basse", "Fichier de rapport"=w712) -> ()  [unwired: 3 in]
                n431 = call "Enregis fichier logbook.vi"("Chaîne"=w703) -> ()  [unwired: 2 in, 1 out]
              }
            }
          }
          event "Test surveillance reg": Value Change {
            n432 = event-data() -> ()  [unwired: 1 in, 6 out]
            n433 = call "Test surveillance reg.vi"() -> ()  [unwired: 12 in]
          }
          event "Début du profil": Value Change {
            # "Bornes du profil"
            n434 = event-data() -> ("NewVal"=w733:timestamp)  [unwired: 1 in, 5 out]
            n435 = local read "Config + programmes"() -> (w731:T3)
            n436 = local read "Val T ini"() -> (w721:dbl)
            n437 = To Double Precision Float(number=w733) -> (double precision float=w722:dbl)
            n438 = Build Array(w722) -> (w727:dbl[])
            n439 = Build Array(w721) -> (w726:dbl[])
            n440 = call "Generer_profil EPC3000.vi"("Temps (s)"=w727, "Num_Prog"=u8 1, "Températures (°C)"=w726, "Programmes et config"=w731) -> ("Temps (s)"=w728:dbl[], "Températures (°C)"=w730:dbl[], "Evennements_sortie"=w729:T15)  [unwired: 1 in]
            n441 = call "Afficher_profil.vi"("Temps (s)"=w728, "Températures (°C)"=w730, "Evennements_entrée"=w729) -> ("Graphe XY"=w724:cluster{"Y":dbl[], "Y":dbl[]}[], "Bornes profil"=w723:T13)  [unwired: 1 in, 2 out]
            n442 = local write "Profil"(w724) -> ()
            n443 = Unbundle By Name(w723) -> ("Temps min"=w735:dbl, "Temps max"=w736:dbl, "Tempé. min"=w737:dbl, "Tempé. max"=w734:dbl)
            n444 = property on="Profil" class="GraphXY (strict)"("XScale.Minimum"=w735, "XScale.Maximum"=w736, "YScale.Minimum"=w737, "YScale.Maximum"=w734) -> (error out=w732:errorcluster)  [unwired: 2 in, 1 out]
            n445 = call <vilib>:"Clear Errors.vi"("error in (no error)"=w732) -> ()  [unwired: 5 in, 2 out]
          }
          event "Onglet_Tinit", "Val T ini": Value Change {
            # "Bornes du profil"
            n446 = event-data() -> ()  [unwired: 1 in, 6 out]
            n447 = Get Date/Time In Seconds() -> (seconds since 1Jan1904=w742:timestamp)
            n448 = global read "Variables glob EUROTHERM.vi" "Ports COM REG run"() -> (w751:refnum<visa-resource-name>[])
            n449 = global read "Variables glob EUROTHERM.vi" "Adresses regs run"() -> (w750:cluster{"Adresses run 1COM reg":u16[]}[])
            n450 = local read "Config + programmes"() -> (w739:T3)
            n451 = local write "Début du profil"(w742) -> ()
            n452 = local read "Onglet_Tinit"() -> (w740:enum32{"Définir Tinit", "Acquérir Tinit"})
            n453 = local read "Val T ini"() -> (w741:dbl)
            n454 = Index Array(array=w751, index=0 ("indice")) -> (element=w744:refnum<visa-resource-name>)
            n455 = Index Array(array=w750, index=0 ("indice")) -> (element=w749:cluster{"Adresses run 1COM reg":u16[]})
            n456 = Unbundle(w749) -> ("Adresses run 1COM reg"=w748:u16[])
            n457 = Index Array(array=w748, index=0 ("indice")) -> (element=w743:u16)
            n458 = call "Mise en forme graphe EPC.vi"("Début du profil"=w742, "Port COM run 1 REG"=w744, "Val T ini en entrée"=w741, "Onglet_Tinit"=w740, "Config + programmes"=w739, "adresse reg"=w743) -> ("Graphe XY"=w752:cluster{"Y":dbl[], "Y":dbl[]}[], "Courbes à afficher"=w738:bool[], "Bornes profil"=w753:T13)  [unwired: 2 in]
            n459 = Unbundle By Name(w753) -> ("Temps min"=w754:dbl, "Temps max"=w755:dbl, "Tempé. min"=w756:dbl, "Tempé. max"=w757:dbl)
            n460 = for {
              tunnel: w738 -> [w758] mode=indexing
              i -> [w759]
              n461 = Increment(x=w759) -> (x+1=w760:i32)
              n462 = property on="Profil" class="GraphXY (strict)"("Active Plot"=w760, "Plot.Visible?"=w758) -> ()  [unwired: 2 in, 2 out]
            }
            n463 = local write "Profil"(w752) -> ()
            n464 = property on="Profil" class="GraphXY (strict)"("XScale.Minimum"=w754, "XScale.Maximum"=w755, "YScale.Minimum"=w756, "YScale.Maximum"=w757) -> ()  [unwired: 2 in, 2 out]
          }
        }
      }
    }
  }
